vi "Process.vi"(8 "error in (no error)":errorcluster, 10 "Event Registration Refnum":refnum<event-registration>, 11 "Test Manager":refnum<class "Basic Test Manager.lvclass">) -> (0 "error out":errorcluster, 3 "Test Manager out":refnum<class "Basic Test Manager.lvclass">)   [LabVIEW 2020, in "Caraya.lvlib" / "Basic Test Manager.lvclass"]
uses:
  Basic Test Manager.lvclass
  Basic Test Manager.lvclass/Basic Test Manager.ctl
  Test Event Storage/Test Event Storage.lvclass
  Test State.ctl
  <vilib>/picture/picture.llb/imagedata.ctl
  Test Result/Test Registration Data.ctl
  Test Result/Test Result.lvclass
  Caraya.lvlib
  Tree Symbol.ctl
  <vilib>/Platform/browser.llb/Open URL in Default Browser (string).vi
  Test Report/Test Report.lvclass
  Test Report.JUnit/Test Report.JUnit.lvclass
  Test Report.Default/Test Report.Default.lvclass
  <userlib>/_OpenG.lib/file/file.llb/openg_file.lvlib
  <userlib>/_OpenG.lib/file/file.llb/Strip Path Extension - String__ogtk.vi
  Test Manager Message/TestManagerMsg.lvclass
  Test Manager Message Assertion/TestManagerMsg.Assertion.lvclass
  Test Manager Message Verbose/TestManagerMsg.Verbose.lvclass
  Test Manager Message KVP/TestManagerMsg.KVP.lvclass
  Test Manager Message Measurement/TestManagerMsg.Measurement.lvclass
  Test Manager Message Test/TestManagerMsg.Test.lvclass
  Test Manager Message Complete Suite/TestManagerMsg.CompleteSuite.lvclass
  Test Report.Event/Test Report.Event.lvclass
  Test Result/Test Node (Extended).ctl
  C:/projects/caraya/src/classes/Test Manager Message/TestManagerMsg.lvclass
  C:/projects/caraya/src/classes/Test Report/Test Report.lvclass
  UI Tab -- enum.ctl
panel:
  out "Processing Time (s)":dbl
  in  "Unknow":bool caption="Unknown"
  out "Pass":bool caption="Passed"
  in  "Fail":bool caption="Failed"
  in  "Hide Passed Tests Checkbox":bool
  out "Error String":string="0 Errors"
  out "Fail String":string="0 Failed"
  out "Pass String":string="0 Passed"
  out "Skip String":string="0 Skipped"
  out "Unknown String":string="0 Unknowns"
  in  "Tab":T1
  out "Report":string
  in  "Tests Tree":string(tree)
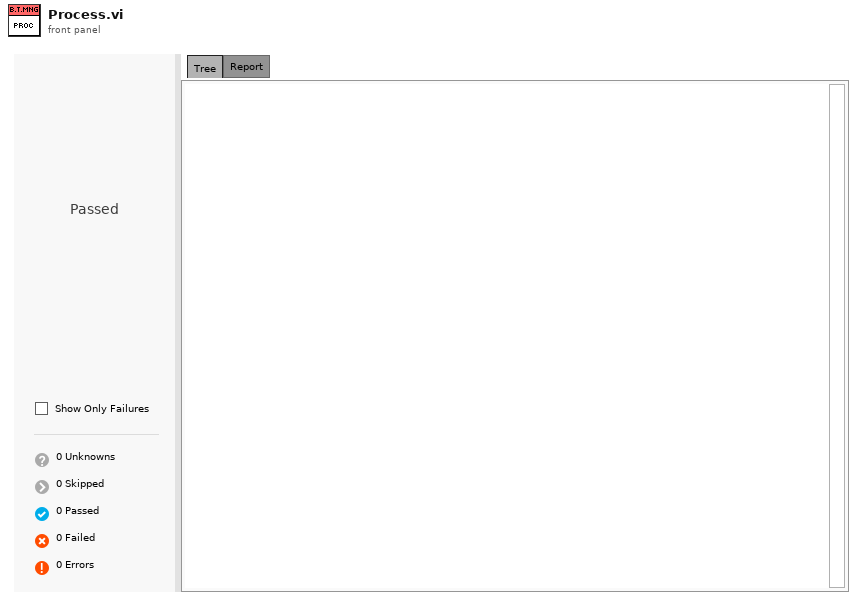
[diagram p1: front panel]
types:
  T1 = typedef "Caraya.lvlib/Basic Test Manager.lvclass/UI Tab -- enum.ctl" = enum32{"Tree", "Report"}
  T2 = enum32{"invalid app kind", "Development System", "Run Time System", "Student Edition", "Embedded LabVIEW", "Evaluation", "Custom"}
  T3 = typedef "Caraya.lvlib/Test Result.lvclass/Test Node (Extended).ctl" = cluster{"Test Registration":T4, "Defined":bool, "Passed":bool, "properties":variant}
  T4 = typedef "Caraya.lvlib/Test Result.lvclass/Test Registration Data.ctl" = cluster{"Name":string, "Call Chain":string[], "Time Stamp":timestamp, "Test ID":string, "Caller ID":string}
  T5 = enum32{"Page Enabled", "Page Disabled", "Page Disabled & Grayed"}
  T6 = enum32{"Invalid", "Standard", "Closed", "Hidden", "Minimized", "Maximized"}
  T7 = typedef "Caraya.lvlib/Basic Test Manager.lvclass/Test State.ctl" = enum16{"Empty", "Unknown", "Fail", "Pass", "Skip", "Error"}
  T8 = cluster{"Core":cluster{"Current VI Reference":refnum<vi>, "Close Panel on Exit?":bool}, "State":T7, "Storage":refnum<class "Test Event Storage.lvclass">, "Argument":variant, "Final State":T7, "Complete":bool, "Last Update":u32, "Running":bool, "Hide Passed Tests":bool, "final error":errorcluster, "Update Delay":u32, "Message":refnum<class "TestManagerMsg.lvclass">, "Tab":T1, "Report Event":refnum<user-event>, "Start Time":timestamp}
  T9 = typedef "LVPoint32TypeDef.ctl" = cluster{"Horizontal":i32, "Vertical":i32}
  T10 = cluster{"Current VI Reference":refnum<vi>, "Close Panel on Exit?":bool}
  T11 = cluster{"Event Registration Refnum":refnum<event-registration>, "local":refnum<event-registration>}
  T12 = typedef "imagedata.ctl" = cluster{"image type":i32, "image depth":i32, "image":u8[], "mask":u8[], "colors":u32[], "Rectangle":cluster{"left":i16, "top":i16, "right":i16, "bottom":i16}}
  T13 = typedef "Caraya.lvlib/Basic Test Manager.lvclass/Tree Symbol.ctl" = enum16{"Empty", "Unknown", "Fail", "Pass", "Skip", "Error", "Fail Node", "Pass Node"}
  T14 = typedef "Caraya.lvlib/Test Result.lvclass/Assert Event Data (Extended).ctl" = cluster{"name":string, "passed":bool, "call-chain":string[], "test-error":errorcluster, "timestamp":timestamp, "assert-id":string, "test-id":string, "time":dbl, "message":string, "properties":variant, "measurements":variant, "user-defined":variant}
  T15 = typedef "Caraya.lvlib/Test Result.lvclass/Test Node.ctl" = cluster{"Test Registration":T4, "Defined":bool, "Passed":bool}
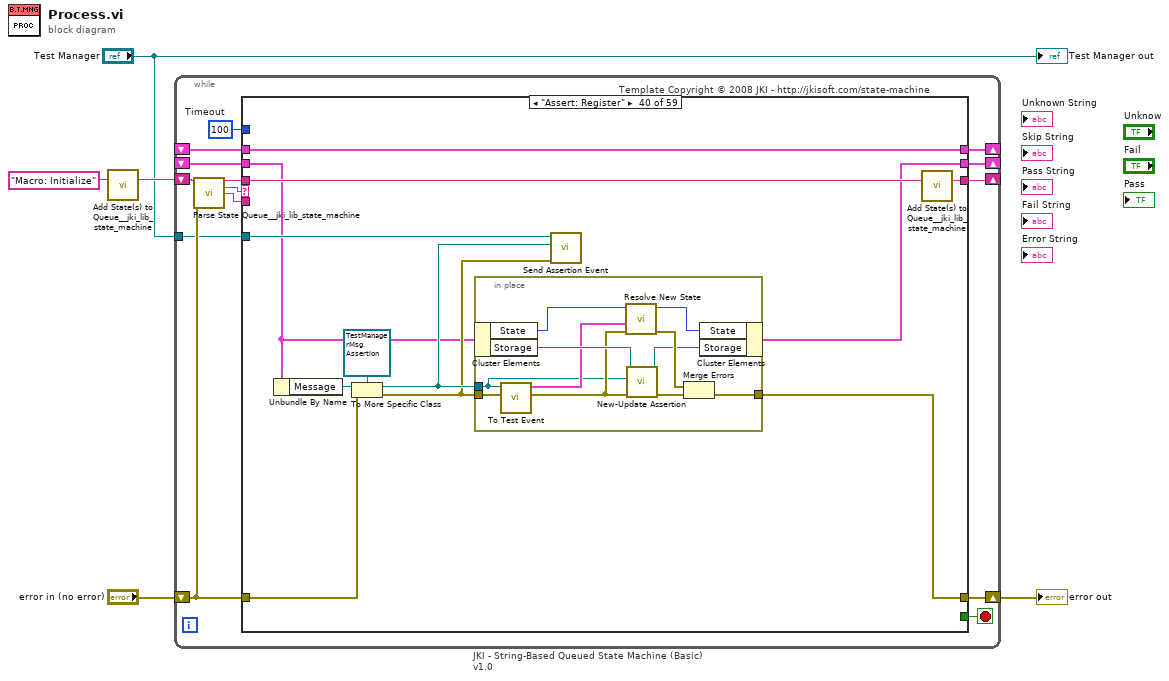
[diagram p0: block diagram]
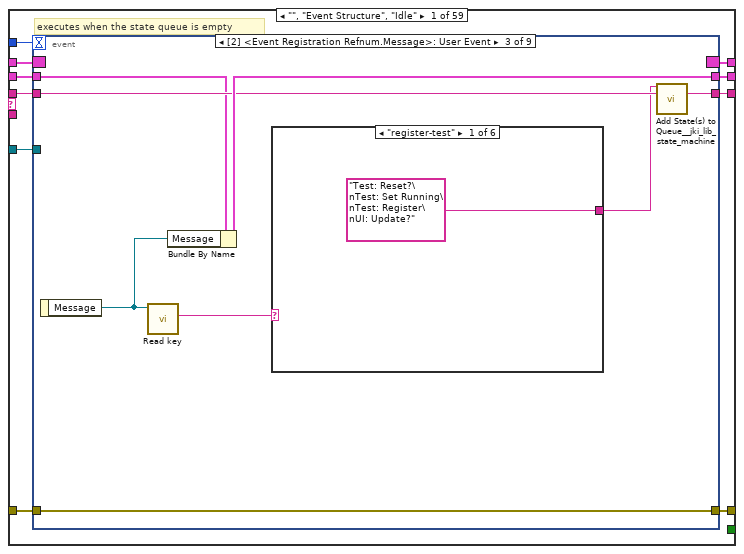
[diagram p2: hidden frame]
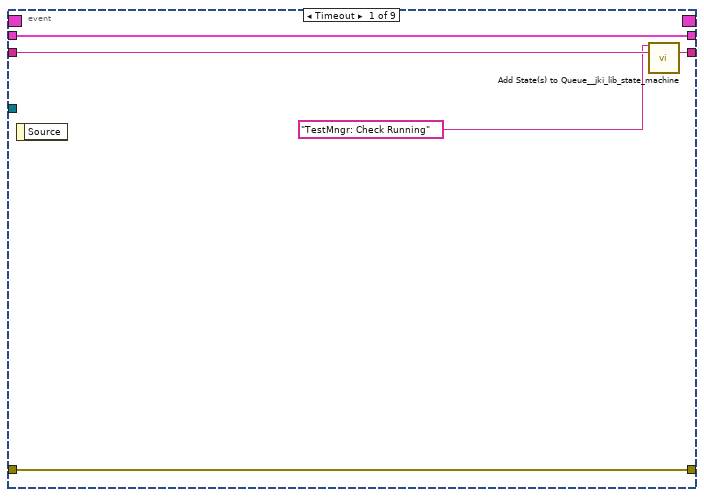
[diagram p3: hidden frame]
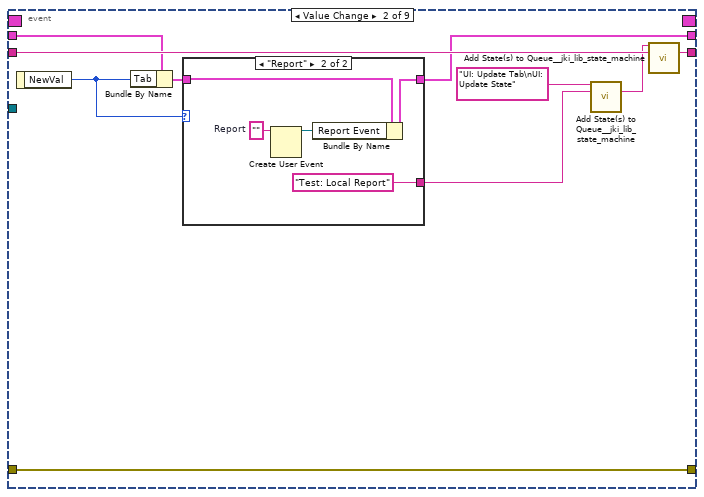
[diagram p4: hidden frame]
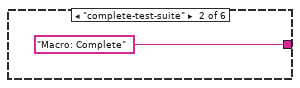
[diagram p6: hidden frame]
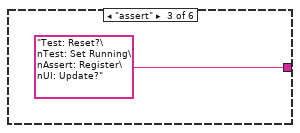
[diagram p7: hidden frame]
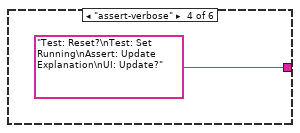
[diagram p8: hidden frame]
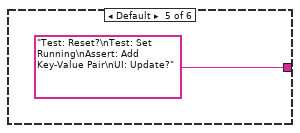
[diagram p9: hidden frame]
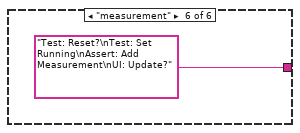
[diagram p10: hidden frame]
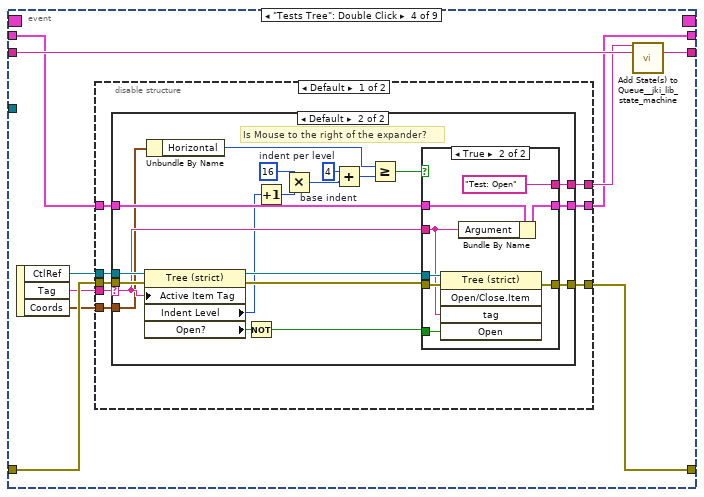
[diagram p11: hidden frame]
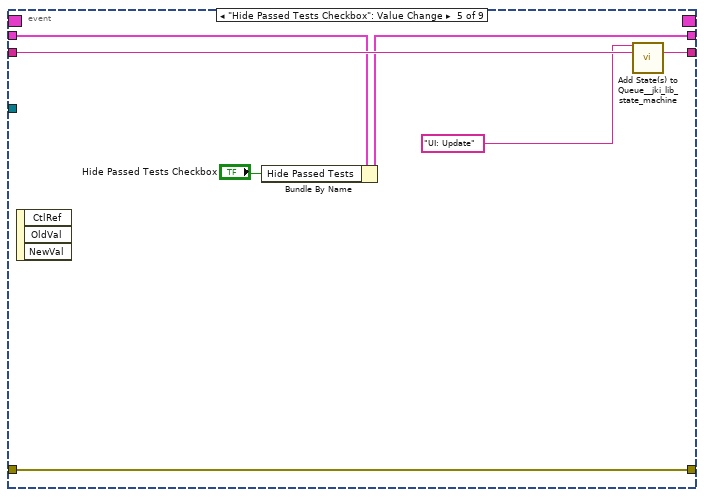
[diagram p15: hidden frame]
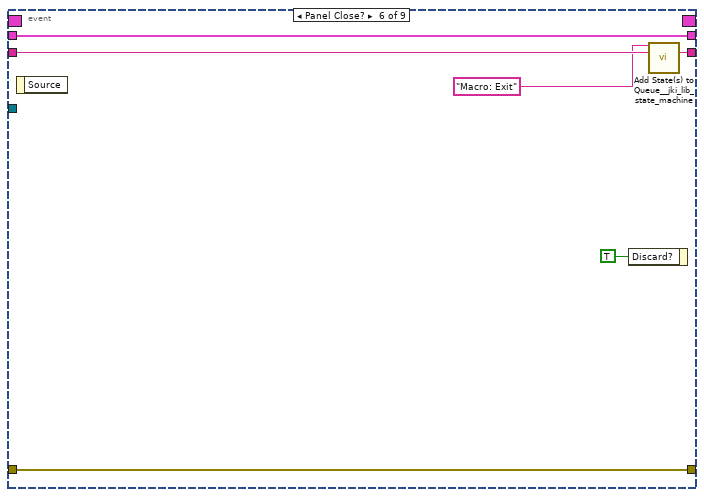
[diagram p16: hidden frame]
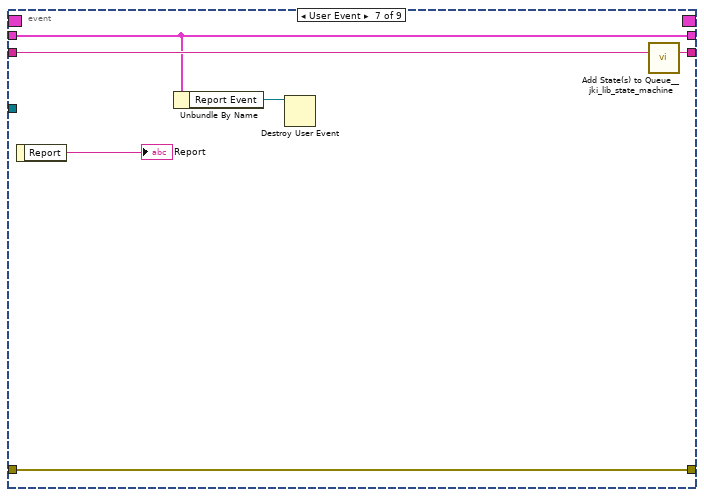
[diagram p17: hidden frame]
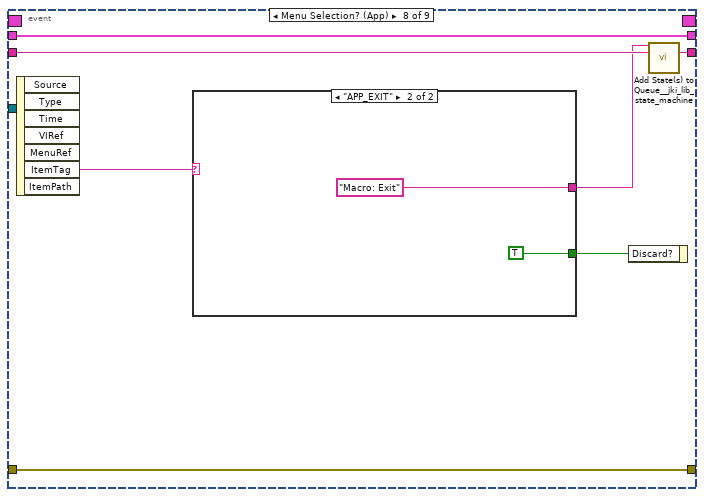
[diagram p18: hidden frame]
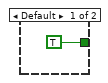
[diagram p19: hidden frame]
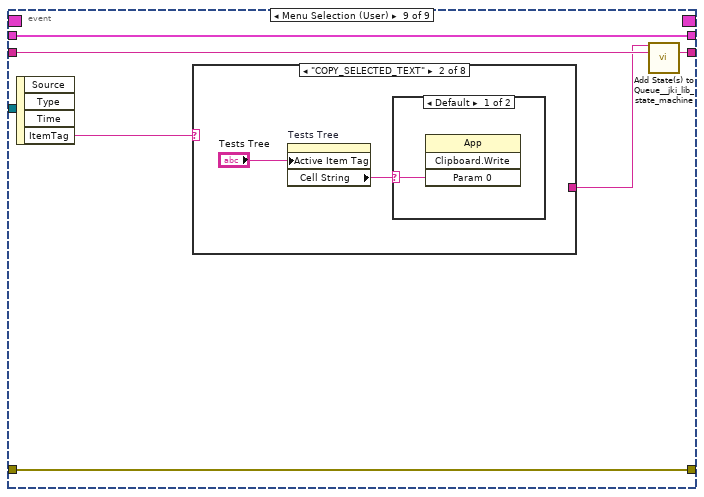
[diagram p20: hidden frame]
diagram:
  n1 = call <vilib>:"Add State(s) to Queue__jki_lib_state_machine.vi"("State(s) in (\"\")"="Macro: Initialize") -> ("States Out"=w5:string)  [unwired: 14 in]
  n2 = while "JKI - String-Based Queued State Machine (Basic) v1.0" {
    shift-right: [w12] -> _
    shift-left: _ -> [w11]
    shift-right: [w15] -> w1
    shift-left: "error in (no error)" -> [w9]
    shift-right: [w14] -> _
    shift-left: w5 -> [w16]
    tunnel: "Test Manager" -> [w7]
    shift-right: [w6] -> _
    shift-left: _ -> [w8]
    stop <- w13 stop-if-true
    w10 = 100  # Timeout
    # "Template Copyright © 2008 JKI - http://jkisoft.com/state-machine"
    n3 = call <vilib>:"Parse State Queue__jki_lib_state_machine.vi"("State Queue"=w16, "Error In (no error)"=w9) -> ("Remaining States"=w18:string, "Current State"=w19:string, "Arguments"=w17:string)  [unwired: 11 in]
    n4 = case shown="\"Assert: Register\"" w19 {
      selector: w19 -> [_ _ w168 _ _ _ _ _ _ _ _ _ _ _ _ _ _ _ _ _ _ _ _ _ _ _ _ _ _ _ _ _ _ _ _ _ _ _ _ _ _ _ _ _ _ _ _ _ _ _ _ _ _ _ _ _ _ _ _]
      tunnel: w18 -> [w29 w165 w172 w190 w202 w213 w219 w224 w240 w251 w256 w265 w270 w277 w283 w296 w304 w316 w329 w339 w345 w357 w367 w385 w391 w411 w463 w505 w539 w556 w574 w607 w613 w619 w625 w631 w637 w649 w654 w666 w687 w712 w734 w755 w771 w776 w796 w807 w809 w856 w883 w892 w899 w909 w921 w943 w957 w987 w1035]
      tunnel: w17 -> [_ _ _ _ _ _ _ _ _ _ _ _ _ _ _ _ _ _ _ _ _ _ _ _ _ _ _ _ w534 w553 w569 _ _ _ _ _ _ _ _ _ _ _ _ _ _ _ _ _ _ _ _ _ _ _ _ _ _ w962 _]
      tunnel: w11 -> [w27 w162 w170 w181 w195 w211 w216 w221 _ w246 w253 w258 w267 w273 w281 w293 w302 w313 w318 w332 w343 w355 w365 w377 w389 w409 w458 w502 w537 w551 w570 w604 w610 w616 w622 w628 w634 w646 w651 w655 w683 w709 w731 w752 w763 w773 w790 w805 w810 w849 w878 w888 w896 w903 w917 w933 w955 w984 w1031]
      tunnel: [w26 w163 w174 w187 errorcluster {"status"=FALSE, "code"=0, "source"=""} ("error out") w208 w215 w222 w242 w247 w254 w263 w268 w275 w279 w294 w300 w314 w327 w337 w341 w354 w363 w383 w388 w408 w459 w503 w535 w552 w571 w605 w611 w617 w623 w629 w635 w647 w652 w663 w678 w702 w735 w753 w767 w774 w794 w802 w811 w845 w881 w890 w897 w907 w918 w931 w948 w985 w1033] -> w15
      tunnel: w9 -> [w25 w163 w173 w187 w198 w208 w215 w222 w242 w248 w254 w263 w268 w275 w280 w294 w301 w314 w327 w337 w342 w353 w364 w383 w387 w407 w461 w503 w536 w549 w572 w605 w611 w617 w623 w629 w635 w647 w652 w660 w684 w704 w728 w753 w768 w774 w793 w803 w813 w846 w881 w890 w897 w907 w919 w928 w952 w977 w1033]
      tunnel: [w28 w164 w171 w189 w201 w212 w218 w223 w244 w250 w255 w264 w269 w276 w282 w295 w303 w315 w328 w338 w344 w356 w366 w384 w390 w410 w462 w504 w538 w555 w573 w606 w612 w618 w624 w630 w636 w648 w653 w665 w688 w714 w737 w754 w770 w775 w795 w806 w814 w855 w882 w891 w898 w908 w920 w942 w956 w986 w1034] -> w14
      tunnel: [_ _ _ _ _ _ TRUE _ _ _ _ _ _ _ _ _ _ _ _ _ _ _ _ _ _ _ _ _ _ _ _ _ _ _ _ _ _ _ _ _ _ _ _ _ _ _ _ _ _ _ _ _ _ _ _ _ _ _ _] -> w13
      tunnel: [w24 w162 w170 w188 w196 w210 w216 w221 w243 w246 w253 w258 w267 w273 w281 w293 w302 w313 w318 w332 w343 w355 w365 w382 w389 w409 w458 w502 w537 w551 w570 w604 w610 w616 w622 w628 w634 w646 w651 w664 w677 w713 w736 w752 w763 w773 w791 w805 w810 w849 w880 w888 w895 w903 w917 w933 w955 w984 w1032] -> w12
      tunnel: w10 -> [w23 _ _ _ _ _ _ _ _ _ _ _ _ _ _ _ _ _ _ _ _ _ _ _ _ _ _ _ _ _ _ _ _ _ _ _ _ _ _ _ _ _ _ _ _ _ _ _ _ _ _ _ _ _ _ _ _ _ _]
      tunnel: w8 -> [w21 w161 w166 w178 w191 w207 w214 w220 w227 w245 w252 _ w266 w271 w278 w289 w298 w311 w317 w330 w340 w352 w362 w373 w386 w406 w457 w501 w533 w548 w568 w603 w608 w614 w620 w626 w632 w638 w650 w659 w682 w705 w726 w751 w756 w772 w785 w797 w808 w844 w873 w884 w893 w900 w911 w939 w944 w959 w1020]
      tunnel: w7 -> [w22 _ _ _ _ _ _ _ _ _ _ _ _ _ _ _ _ _ _ w333 _ _ _ _ _ _ _ _ _ _ _ _ _ _ _ _ _ _ _ w658 w681 w711 w733 _ _ _ w784 _ w812 _ _ _ _ w904 w915 w927 w953 w970 _]
      tunnel: [w20 w161 w166 w178 w191 w207 w214 w220 w227 w245 w252 w261 w266 w271 w278 w289 w298 w311 w317 w330 w340 w352 w362 w373 w386 w406 w457 w501 w533 w548 w568 w603 w608 w614 w620 w626 w632 w638 w650 w659 w682 w705 w726 w751 w756 w772 w785 w797 w808 w844 w873 w884 w893 w900 w911 w939 w944 w959 w1020] -> w6
      frame "", "Event Structure", "Idle" {
        # "executes when the state queue is empty"
        n5 = event shown="[2] <Event Registration Refnum.Message>: User Event" {
          selector: w21 -> [_ _ _ _ _ _ _ _ _]
          dyn-events: [_ _ _ _ _ _ _ _ _] -> w20
          timeout: w23 -> [_ _ _ _ _ _ _ _ _]
          tunnel: w29 -> [w34 w44 w54 w73 w122 w129 w135 w142 w151]
          tunnel: [w33 w43 w55 w74 w123 w128 w134 w141 w150] -> w28
          tunnel: w27 -> [w31 w41 w52 w68 w119 w126 w131 w139 w148]
          tunnel: [w32 w42 w58 w71 w120 w127 w133 w140 w149] -> w26
          tunnel: w25 -> [w32 w42 w58 w70 w120 w127 w133 w140 w149]
          tunnel: [w31 w35 w56 w69 w118 w126 w131 w139 w148] -> w24
          tunnel: w22 -> [_ _ _ _ _ _ _ _ _]
          event Timeout {
            n6 = event-data() -> ()  [unwired: 1 in, 1 out]
            n7 = call <vilib>:"Add State(s) to Queue__jki_lib_state_machine.vi"("State(s) in Front (\"\")"="TestMngr: Check Running", "State(s) in (\"\")"=w34) -> ("States Out"=w33:string)  [unwired: 13 in]
          }
          event Value Change {
            n8 = event-data() -> ("NewVal"=w38:T1)  [unwired: 1 in]
            n9 = Bundle By Name(cluster=w41, "Tab"=w38) -> (w36:T8)
            n10 = case shown="\"Report\"" w38 {
              tunnel: [_ "Test: Local Report"] -> w37
              tunnel: w36 -> [w45 w49]
              tunnel: [w45 w48] -> w35
              frame Default {
              }
              frame "Report" {
                w47 = ""  # Report
                n11 = Create User Event(user event datatype=w47) -> (user event=w46:refnum<user-event>)  [unwired: 1 in, 1 out]
                n12 = Bundle By Name(cluster=w49, "Report Event"=w46) -> (w48:T8)
              }
            }
            n13 = call <vilib>:"Add State(s) to Queue__jki_lib_state_machine.vi"("State(s) in Front (\"\")"="UI: Update Tab\nUI: Update State", "State(s) in (\"\")"=w37) -> ("States Out"=w39:string)  [unwired: 13 in]
            n14 = call <vilib>:"Add State(s) to Queue__jki_lib_state_machine.vi"("State(s) in Front (\"\")"=w39, "State(s) in (\"\")"=w44) -> ("States Out"=w43:string)  [unwired: 13 in]
          }
          event User Event {
            n15 = event-data() -> ("Message"=w57:refnum<class "TestManagerMsg.lvclass">)  [unwired: 1 in]
            n16 = call "Read key.vi"("TestManagerMsg in"=w57) -> ("key"=w51:string)  [unwired: 9 in, 1 out]
            n17 = Bundle By Name(cluster=w52, "Message"=w57) -> (w56:T8)
            n18 = case shown="\"register-test\"" w51 {
              tunnel: ["Test: Reset?\nTest: Set Running\nTest: Register\nUI: Update?" "Macro: Complete" "Test: Reset?\nTest: Set Running\nAssert: Register\nUI: Update?" "Test: Reset?\nTest: Set Running\nAssert: Update Explanation\nUI: Update?" "Test: Reset?\nTest: Set Running\nAssert: Add Key-Value Pair\nUI: Update?" "Test: Reset?\nTest: Set Running\nAssert: Add Measurement\nUI: Update?"] -> w53
              frame "register-test" {
              }
              frame "complete-test-suite" {
              }
              frame "assert" {
              }
              frame "assert-verbose" {
              }
              frame Default {
              }
              frame "measurement" {
              }
            }
            n19 = call <vilib>:"Add State(s) to Queue__jki_lib_state_machine.vi"("State(s) in Front (\"\")"=w53, "State(s) in (\"\")"=w54) -> ("States Out"=w55:string)  [unwired: 13 in]
          }
          event "Tests Tree": Double Click {
            n20 = event-data() -> ("CtlRef"=w66:refnum<vi>, "Tag"=w67:string, "Coords"=w65:T9)  [unwired: 1 in]
            n21 = disable-structure shown="Default" {
              disable-tunnel: [w82 _] -> w72
              disable-tunnel: [w81 w115] -> w71
              disable-tunnel: w70 -> [w80 w115]
              disable-tunnel: [w79 w116] -> w69
              disable-tunnel: w68 -> [w78 w116]
              disable-tunnel: w67 -> [w77 _]
              disable-tunnel: w66 -> [w76 _]
              disable-tunnel: w65 -> [w75 _]
              frame condition #0 (active) {
                n22 = case shown="Default" w77 {
                  selector: w77 -> [_ w99]
                  tunnel: [_ w104] -> w82
                  tunnel: [w83 w86] -> w81
                  tunnel: w76 -> [_ w103]
                  tunnel: w80 -> [w83 w102]
                  tunnel: w78 -> [w84 w101]
                  tunnel: [w84 w100] -> w79
                  tunnel: w75 -> [_ w90]
                  frame "" {
                  }
                  frame Default {
                    w93 = 16  # indent per level
                    w92 = 4  # base indent
                    # "Is Mouse to the right of the expander?"
                    n23 = property class="Tree (strict)"(reference=w103, error in=w102, "Active Item Tag"=w99) -> (reference out=w98:refnum<vi>, error out=w97:errorcluster, "Indent Level"=w95:i32, "Open?"=w96:bool)
                    n24 = Unbundle By Name(w90) -> ("Horizontal"=w88:i32)
                    n25 = Not(x=w96) -> (.not. x?=w85:bool)
                    n26 = Increment(x=w95) -> (x+1=w94:i32)
                    n27 = Multiply(x=w93, y=w94) -> (x*y=w91:i32)
                    n28 = Add(x=w92, y=w91) -> (x+y=w87:i32)
                    n29 = Greater Or Equal?(x=w88, y=w87) -> (x >= y?=w89:bool)
                    n30 = case shown="True" w89 {
                      tunnel: [_ "Test: Open" ("State(s) in Front (\"\")")] -> w104
                      tunnel: w101 -> [w106 w113]
                      tunnel: [w106 w112] -> w100
                      tunnel: w99 -> [_ w108]
                      tunnel: [w105 w110] -> w86
                      tunnel: w98 -> [_ w109]
                      tunnel: w97 -> [w105 w111]
                      tunnel: w85 -> [_ w107]
                      frame False {
                      }
                      frame True {
                        n31 = invoke class="Tree (strict)" method="Open/Close.Item"(reference=w109, error in=w111, "tag"=w108, "Open"=w107) -> (error out=w110:errorcluster)  [unwired: 1 in, 4 out]
                        n32 = Bundle By Name(cluster=w113, "Argument"=w108) -> (w112:T8)
                      }
                    }
                  }
                }
              }
              frame condition #1 {
              }
            }
            n33 = call <vilib>:"Add State(s) to Queue__jki_lib_state_machine.vi"("State(s) in Front (\"\")"=w72, "State(s) in (\"\")"=w73) -> ("States Out"=w74:string)  [unwired: 13 in]
          }
          event "Hide Passed Tests Checkbox": Value Change {
            n34 = event-data() -> ()  [unwired: 1 in, 3 out]
            n35 = Bundle By Name(cluster=w119, "Hide Passed Tests"="Hide Passed Tests Checkbox") -> (w118:T8)
            n36 = call <vilib>:"Add State(s) to Queue__jki_lib_state_machine.vi"("State(s) in Front (\"\")"="UI: Update" ("State(s) in Front (\"\")"), "State(s) in (\"\")"=w122) -> ("States Out"=w123:string)  [unwired: 13 in]
          }
          event Panel Close? {
            n37 = event-data() -> ()  [unwired: 1 in, 1 out]
            n38 = event-data("Discard?"=TRUE) -> ()  [unwired: 1 in, 1 out]
            n39 = call <vilib>:"Add State(s) to Queue__jki_lib_state_machine.vi"("State(s) in Front (\"\")"="Macro: Exit", "State(s) in (\"\")"=w129) -> ("States Out"=w128:string)  [unwired: 13 in]
          }
          event User Event {
            n40 = event-data() -> ("Report"=→"Report":string)  [unwired: 1 in]
            n41 = Unbundle By Name(w131) -> ("Report Event"=w130:refnum<user-event>)
            n42 = Destroy User Event(user event=w130) -> ()  [unwired: 1 in, 1 out]
            n43 = call <vilib>:"Add State(s) to Queue__jki_lib_state_machine.vi"("State(s) in (\"\")"=w135) -> ("States Out"=w134:string)  [unwired: 14 in]
          }
          event Menu Selection? (App) {
            n44 = event-data() -> ("ItemTag"=w137:string)  [unwired: 1 in, 6 out]
            n45 = case shown="\"APP_EXIT\"" w137 {
              tunnel: [_ "Macro: Exit"] -> w138
              tunnel: [TRUE TRUE] -> w136
              frame Default {
              }
              frame "APP_EXIT" {
              }
            }
            n46 = event-data("Discard?"=w136) -> ()  [unwired: 1 in, 1 out]
            n47 = call <vilib>:"Add State(s) to Queue__jki_lib_state_machine.vi"("State(s) in Front (\"\")"=w138, "State(s) in (\"\")"=w142) -> ("States Out"=w141:string)  [unwired: 13 in]
          }
          event Menu Selection (User) {
            n48 = event-data() -> ("ItemTag"=w146:string)  [unwired: 1 in, 3 out]
            n49 = case shown="\"COPY_SELECTED_TEXT\"" w146 {
              tunnel: [_ _ "Macro: Export" "Macro: Export JUnit" "Macro: Rerun" "UI: About" "UI: Homepage" "Macro: Exit"] -> w147
              frame Default {
              }
              frame "COPY_SELECTED_TEXT" {
                n50 = property on="Tests Tree" class="Tree (strict)"("Active Item Tag"="Tests Tree") -> ("Cell String"=w152:string)  [unwired: 2 in, 2 out]
                n51 = case shown="Default" w152 {
                  selector: w152 -> [w154 _]
                  frame Default {
                    n52 = invoke class="App" method="Clipboard.Write"("Param 0"=w154) -> ()  [unwired: 3 in, 4 out]
                  }
                  frame "" {
                  }
                }
              }
              frame "FILE_EXPORT" {
              }
              frame "FILE_EXPORT_JUNIT" {
              }
              frame "TEST_RERUN" {
              }
              frame "HELP_ABOUT" {
              }
              frame "HOME_PAGE" {
              }
              frame "FILE_CLOSE" {
              }
            }
            n53 = call <vilib>:"Add State(s) to Queue__jki_lib_state_machine.vi"("State(s) in Front (\"\")"=w147, "State(s) in (\"\")"=w151) -> ("States Out"=w150:string)  [unwired: 13 in]
          }
        }
      }
      frame "---------- Core ----------" {
        # "Do not put any code in this frame.\n(it is a separator no-op)"
        n54 = call <vilib>:"Add State(s) to Queue__jki_lib_state_machine.vi"("State(s) in (\"\")"=w165) -> ("States Out"=w164:string)  [unwired: 14 in]
      }
      frame Default {
        # "Current State"
        # "Do not delete, rename, or modify this frame.\n(this is used to capture unhandled states and typos)"
        # "Handle mistyped state name (developer tool)"
        n55 = Format Into String(format string="Software Exception: Unhandled State \"%s\"." ("message"), error in=w173, w168) -> (resulting string=w176:string, error out=w175:errorcluster)  [unwired: 1 in]
        n56 = call <vilib>:"Error Cluster From Error Code.vi"("show call chain? (False)"=TRUE, "error in (no error)"=w175, "error message (\"\")"=w176, "error code (0)"=7000) -> ("error out"=w174:errorcluster)  [unwired: 5 in]
        n57 = call <vilib>:"Add State(s) to Queue__jki_lib_state_machine.vi"("State(s) in (\"\")"=w172) -> ("States Out"=w171:string)  [unwired: 14 in]
      }
      frame "Initialize Core Data" {
        # "Do not delete, rename, or modify this frame.\n(this is used to determine panel behavior on exit)"
        # "originally closed?"
        # "exe?"
        # "If panel starts closed or is an EXE, then close it when we exit"
        n58 = stacked-sequence {
          frame #0 {
            # "Do not delete. This reference forces\nFront Panel in memory in EXE."
            n59 = control-ref of="Test Manager"() -> ()  [unwired: 1 out]
          }
        }
        n60 = property class="VI"() -> ("Front Panel.Open"=w186:bool)  [unwired: 2 in, 2 out]
        n61 = property class="App"() -> ("App.Kind"=w185:T2)  [unwired: 2 in, 2 out]
        n62 = control-ref of="Current VI Reference"() -> (w179:refnum<vi>)
        n63 = Not(x=w186) -> (.not. x?=w183:bool)
        n64 = Equal?(x=w185, y=T2."Run Time System" ("Application:Kind")) -> (x = y?=w182:bool)
        n65 = Or(x=w183, y=w182) -> (x .or. y?=w180:bool)
        n66 = Bundle By Name(cluster=w181, "Core.Current VI Reference"=w179, "Core.Close Panel on Exit?"=w180) -> (w188:T8)
        n67 = call <vilib>:"Add State(s) to Queue__jki_lib_state_machine.vi"("State(s) in (\"\")"=w190) -> ("States Out"=w189:string)  [unwired: 14 in]
      }
      frame "Error Handler" {
        # "Clear error"
        # "Handle any errors here.\nYou can also output any states to clean-up after errors occur"
        n68 = Unbundle By Name(w198) -> ("code"=w199:i32)
        n69 = case shown="Default" w199 {
          tunnel: w198 -> [w203 w204 w206]
          tunnel: [w203 w204 w205] -> w193
          frame 7000..7999 {
            # "All Caraya Error range"
          }
          frame 1 {
          }
          frame Default {
            # "Unhandled Error -- Display it"
            n70 = call <vilib>:"General Error Handler.vi"("error in (no error)"=w206) -> ("error out"=w205:errorcluster)  [unwired: 10 in, 4 out]
          }
        }
        n71 = Unbundle By Name(w195) -> ("final error"=w194:errorcluster)
        n72 = Merge Errors(w194, w193) -> (w192:errorcluster)
        n73 = Bundle By Name(cluster=w195, "final error"=w192) -> (w196:T8)
        n74 = call <vilib>:"Add State(s) to Queue__jki_lib_state_machine.vi"("State(s) in Front (\"\")"="/* Post Error States", "State(s) in (\"\")"=w202) -> ("States Out"=w201:string)  [unwired: 13 in]
      }
      frame "Reset Final Error" {
        # "Clear error"
        n75 = Bundle By Name(cluster=w211, "final error"=errorcluster {"status"=FALSE, "code"=0, "source"=""} ("error out")) -> (w210:T8)
        n76 = call <vilib>:"Add State(s) to Queue__jki_lib_state_machine.vi"("State(s) in (\"\")"=w213) -> ("States Out"=w212:string)  [unwired: 14 in]
      }
      frame "Exit" {
        # "Do not put any code in this frame.\n(No errors that occur here will be handled.)"
        n77 = call <vilib>:"Add State(s) to Queue__jki_lib_state_machine.vi"("State(s) in (\"\")"=w219) -> ("States Out"=w218:string)  [unwired: 14 in]
      }
      frame "---------- Data ----------" {
        # "Do not put any code in this frame.\n(It is a separator no-op. You can make a copy of this frame to create a new Data frame)"
        n78 = call <vilib>:"Add State(s) to Queue__jki_lib_state_machine.vi"("State(s) in (\"\")"=w224) -> ("States Out"=w223:string)  [unwired: 14 in]
      }
      frame "Data: Initialize" {
        w225 = timestamp(0 s since 1904-01-01)  # Start Time
        w226 = refnum<user-event> refnum  # Report Event
        w229 = refnum<class "TestManagerMsg.lvclass"> refnum  # Message
        w230 = u32 100  # Update Delay
        w231 = errorcluster {"status"=FALSE, "code"=0, "source"=""}  # final error
        w232 = FALSE  # Hide Passed Tests
        w233 = FALSE  # Running
        w234 = u32 0  # Last Update
        w235 = FALSE  # Complete
        w236 = Test_State."Unknown"  # Final State
        w237 = variant  # Argument
        w239 = Test_State."Unknown"  # State
        w238 = refnum<class "Test Event Storage.lvclass"> refnum  # Storage
        w241 = T10 {"Current VI Reference"=refnum, "Close Panel on Exit?"=FALSE}  # Core
        # "Initialize the shift-register data, here.\n(data names are defined by what you wire into the bundle function)"
        n79 = Bundle("Core"=w241, "State"=w239, "Storage"=w238, "Argument"=w237, "Final State"=w236, "Complete"=w235, "Last Update"=w234, "Running"=w233, "Hide Passed Tests"=w232, "final error"=w231, "Update Delay"=w230, "Message"=w229, "Tab"="Tab", "Report Event"=w226, "Start Time"=w225) -> (w243:T8)  [unwired: 1 in]
        n80 = call <vilib>:"Add State(s) to Queue__jki_lib_state_machine.vi"("State(s) in (\"\")"=w240) -> ("States Out"=w244:string)  [unwired: 14 in]
      }
      frame "Data: Cleanup" {
        # "Cleanup any data and references, here.\n(this is called automatically, by the Macro: Exit)"
        n81 = Unbundle By Name(w246) -> ("Core.Current VI Reference"=w249:refnum<vi>)
        n82 = Close Reference(reference=w249, error in (no error)=w248) -> (error out=w247:errorcluster)
        n83 = call <vilib>:"Add State(s) to Queue__jki_lib_state_machine.vi"("State(s) in (\"\")"=w251) -> ("States Out"=w250:string)  [unwired: 14 in]
      }
      frame "---------- Event ----------" {
        # "Do not put any code in this frame.\n(It is a separator no-op. You can make a copy of this frame to create a new UI frame)"
        n84 = call <vilib>:"Add State(s) to Queue__jki_lib_state_machine.vi"("State(s) in (\"\")"=w256) -> ("States Out"=w255:string)  [unwired: 14 in]
      }
      frame "Event: Register" {
        w260 = refnum<event-registration> refnum  # local
        n85 = Unbundle By Name(w258) -> ("Report Event"=w257:refnum<user-event>)
        n86 = register-events(reference=w260, w257) -> (reference out=w262:refnum<event-registration>)  [unwired: 1 in, 1 out]
        n87 = Bundle("Event Registration Refnum"="Event Registration Refnum", "local"=w262) -> (w261:T11)  [unwired: 1 in]
        n88 = call <vilib>:"Add State(s) to Queue__jki_lib_state_machine.vi"("State(s) in (\"\")"=w265) -> ("States Out"=w264:string)  [unwired: 14 in]
      }
      frame "---------- UI ----------" {
        # "Do not put any code in this frame.\n(It is a separator no-op. You can make a copy of this frame to create a new UI frame)"
        n89 = call <vilib>:"Add State(s) to Queue__jki_lib_state_machine.vi"("State(s) in (\"\")"=w270) -> ("States Out"=w269:string)  [unwired: 14 in]
      }
      frame "UI: Initialize" {
        # "Initialize the User Interface, here.\n(this is called automatically, by the Macro: Init)"
        n90 = Unbundle By Name(w273) -> ("Hide Passed Tests"=w272:bool)
        n91 = local write "Hide Passed Tests Checkbox"(w272) -> ()
        n92 = call <vilib>:"Add State(s) to Queue__jki_lib_state_machine.vi"("State(s) in Front (\"\")"="//UI: Defer Updates >> True\nUI: Initialize Icons\nUI: Clear\nUI: Update Title\nUI: Update State\nUI: Set Last Update\n//UI: Defer Updates >> False", "State(s) in (\"\")"=w277) -> ("States Out"=w276:string)  [unwired: 13 in]
      }
      frame "UI: Update Title" {
        n93 = disable-structure shown="Default" {
          disable-tunnel: w280 -> [w285 w288]
          disable-tunnel: [w284 w288] -> w279
          frame condition #0 (active) {
            n94 = control-ref of="This VI"() -> (w287:refnum<vi>)
            n95 = call "Get Library Info.vi"("error in (no error)"=w285) -> ("error out"=w284:errorcluster, "Name"=w286:string)  [unwired: 6 in, 3 out]
            n96 = property class="VI"(reference=w287, "Front Panel.Title"=w286) -> ()  [unwired: 1 in, 2 out]
          }
          frame condition #1 {
          }
        }
        n97 = call <vilib>:"Add State(s) to Queue__jki_lib_state_machine.vi"("State(s) in (\"\")"=w283) -> ("States Out"=w282:string)  [unwired: 14 in]
      }
      frame "UI: Update Tab" {
        n98 = Unbundle By Name(w293) -> ("Tab"=w292:T1)
        n99 = Type Cast(type=0, x=w292) -> (*(type *) &x=w290:i32)
        n100 = case shown="1" w290 {
          frame Default {
          }
          frame 1 {
            # "Report Tab.\nIf no report, produce it."
            n101 = local write "Report"("Refreshing report.\nPlease wait... " ("Report")) -> ()
          }
        }
        n102 = call <vilib>:"Add State(s) to Queue__jki_lib_state_machine.vi"("State(s) in (\"\")"=w296) -> ("States Out"=w295:string)  [unwired: 14 in]
      }
      frame "UI: Clear" {
        # "Initialize the User Interface, here.\n(this is called automatically, by the Macro: Init)"
        n103 = disable-structure shown="Default" {
          disable-tunnel: w301 -> [w307 w310]
          disable-tunnel: [w306 w310] -> w300
          frame condition #0 (active) {
            n104 = control-ref of="Tests Tree"() -> (w308:refnum<vi>)
            n105 = property on="Report" class="Str"("Text.FontName"="Courier New" ("Text.Font:Name")) -> ()  [unwired: 2 in, 2 out]
            n106 = invoke class="Tree (strict)" method="Edit Tree Items.Delete"(reference=w308, error in=w307, "Delete Children"=TRUE ("Delete Children?")) -> (error out=w306:errorcluster)  [unwired: 2 in, 4 out]
          }
          frame condition #1 {
          }
        }
        n107 = local write "Report"("") -> ()
        n108 = call <vilib>:"Add State(s) to Queue__jki_lib_state_machine.vi"("State(s) in (\"\")"=w304) -> ("States Out"=w303:string)  [unwired: 14 in]
      }
      frame "UI: Update" {
        n109 = call <vilib>:"Add State(s) to Queue__jki_lib_state_machine.vi"("State(s) in Front (\"\")"="UI: Defer Updates >> True\nUI: Clear\nUI: Update Asserts\nUI: Update Counts\nUI: Update State\nUI: Set Last Update\nUI: Defer Updates >> False", "State(s) in (\"\")"=w316) -> ("States Out"=w315:string)  [unwired: 13 in]
      }
      frame "UI: Update?" {
        n110 = Unbundle By Name(w318) -> ("Last Update"=w323:u32, "Update Delay"=w320:u32)
        n111 = Tick Count (ms)() -> (millisecond timer value=w324:u32)
        n112 = Subtract(x=w324, y=w323) -> (x-y=w322:u32)
        n113 = Greater?(x=w322, y=w320) -> (0:w319:bool)
        n114 = Select(t="UI: Update" ("State(s) in Front (\"\")"), s=w319, f="") -> (s? t:f=w321:string)
        n115 = call <vilib>:"Add State(s) to Queue__jki_lib_state_machine.vi"("State(s) in Front (\"\")"=w321, "State(s) in (\"\")"=w329) -> ("States Out"=w328:string)  [unwired: 13 in]
      }
      frame "UI: Open" {
        n116 = Unbundle By Name(w333) -> ("Interactive"=w331:bool)
        n117 = Select(t="UI: Front Panel State >> Open" ("State(s) in Front (\"\")"), s=w331, f="") -> (s? t:f=w334:string)
        n118 = call <vilib>:"Add State(s) to Queue__jki_lib_state_machine.vi"("State(s) in Front (\"\")"=w334, "State(s) in (\"\")"=w339) -> ("States Out"=w338:string)  [unwired: 13 in]
      }
      frame "UI: About" {
        n119 = disable-structure shown="Default" {
          disable-tunnel: w342 -> [w349 w351]
          disable-tunnel: [w348 w351] -> w341
          frame condition #0 (active) {
            n120 = vi-ref "About.vi"() -> (w350:refnum<vi>)
            n121 = invoke class="VI" method="Run VI"(reference=w350, error in=w349, "Wait until done"=FALSE ("Wait Until Done"), "Auto Dispose Ref"=TRUE ("Auto Dispose Reference")) -> (error out=w348:errorcluster)  [unwired: 1 in, 4 out]
          }
          frame condition #1 {
          }
        }
        n122 = call <vilib>:"Add State(s) to Queue__jki_lib_state_machine.vi"("State(s) in (\"\")"=w345) -> ("States Out"=w344:string)  [unwired: 14 in]
      }
      frame "UI: Homepage" {
        n123 = disable-structure shown="Default" {
          disable-tunnel: [w360 w361] -> w354
          disable-tunnel: w353 -> [w359 w361]
          frame condition #0 (active) {
            n124 = call-poly <vilib>:"Open URL in Default Browser.vi"("error in (no error)"=w359, "URL"="https://github.com/JKISoftware/Caraya") -> ("error out"=w360:errorcluster)  [unwired: 4 in, 1 out]
          }
          frame condition #1 {
          }
        }
        n125 = call <vilib>:"Add State(s) to Queue__jki_lib_state_machine.vi"("State(s) in (\"\")"=w357) -> ("States Out"=w356:string)  [unwired: 14 in]
      }
      frame "UI: Notify" {
        n126 = disable-structure shown="Default" {
          disable-tunnel: w364 -> [w369 w372]
          disable-tunnel: [w368 w372] -> w363
          frame condition #0 (active) {
            n127 = control-ref of="This VI"() -> (w371:refnum<vi>)
            n128 = property class="VI"(reference=w371, error in=w369, "Front Panel.IsFrontmost"=TRUE ("Front Panel Window:Is Frontmost")) -> (error out=w368:errorcluster)  [unwired: 1 out]
          }
          frame condition #1 {
          }
        }
        n129 = call <vilib>:"Add State(s) to Queue__jki_lib_state_machine.vi"("State(s) in (\"\")"=w367) -> ("States Out"=w366:string)  [unwired: 14 in]
      }
      frame "UI: Set Last Update" {
        # "Geometric progression of update refreshes.\nThe more tests there are, the longer the app\nwaits before refreshing the tree.\n\nThis is not a solid solution, but it will mitigate\nthe lagging for large number of tests in interactive mode."
        n130 = Unbundle By Name(w377) -> ("Update Delay"=w376:u32)
        n131 = Tick Count (ms)() -> (millisecond timer value=w381:u32)
        n132 = Multiply(x=2.0, y=w376) -> (x*y=w379:dbl)
        n133 = To Unsigned Long Integer(number=w379) -> (unsigned 32bit integer=w378:u32)
        n134 = Select(t=w378, s=TRUE, f=w376) -> (s? t:f=w375:u32)
        n135 = Bundle By Name(cluster=w377, "Last Update"=w381, "Update Delay"=w375) -> (w382:T8)
        n136 = call <vilib>:"Add State(s) to Queue__jki_lib_state_machine.vi"("State(s) in (\"\")"=w385) -> ("States Out"=w384:string)  [unwired: 14 in]
      }
      frame "UI: Initialize Icons" {
        # "Initialize the User Interface, here.\n(this is called automatically, by the Macro: Init)"
        n137 = disable-structure shown="Default" {
          disable-tunnel: [w394 w405] -> w388
          disable-tunnel: w387 -> [w393 w405]
          frame condition #0 (active) {
            w392 = cluster{"Image":T12, "Index":T13}[] [{"Image"={"image type"=0, "image depth"=32, "image"=array[1024 elements], "mask"=[255, 255, 255, 255, 255, 255, 255, 255, 255, 255, 255, 255, 255, 255, 255, 255, 255, 255, 255, 255, 255, 255, 255, 255, 255, 255, 255, 255, 255, 255, 255, 255], "colors"=[], "Rectangle"={"left"=0, "top"=0, "right"=16, "bottom"=16}}, "Index"=enum."Unknown"}, {"Image"={"image type"=0, "image depth"=32, "image"=array[1024 elements], "mask"=[255, 255, 255, 255, 255, 255, 255, 255, 255, 255, 255, 255, 255, 255, 255, 255, 255, 255, 255, 255, 255, 255, 255, 255, 255, 255, 255, 255, 255, 255, 255, 255], "colors"=[], "Rectangle"={"left"=0, "top"=0, "right"=16, "bottom"=16}}, "Index"=enum."Fail"}, {"Image"={"image type"=0, "image depth"=32, "image"=array[1024 elements], "mask"=[255, 255, 255, 255, 255, 255, 255, 255, 255, 255, 255, 255, 255, 255, 255, 255, 255, 255, 255, 255, 255, 255, 255, 255, 255, 255, 255, 255, 255, 255, 255, 255], "colors"=[], "Rectangle"={"left"=0, "top"=0, "right"=16, "bottom"=16}}, "Index"=enum."Pass"}, {"Image"={"image type"=0, "image depth"=32, "image"=array[1024 elements], "mask"=[255, 255, 255, 255, 255, 255, 255, 255, 255, 255, 255, 255, 255, 255, 255, 255, 255, 255, 255, 255, 255, 255, 255, 255, 255, 255, 255, 255, 255, 255, 255, 255], "colors"=[], "Rectangle"={"left"=0, "top"=0, "right"=16, "bottom"=16}}, "Index"=enum."Skip"}, {"Image"={"image type"=0, "image depth"=32, "image"=array[1024 elements], "mask"=[255, 255, 255, 255, 255, 255, 255, 255, 255, 255, 255, 255, 255, 255, 255, 255, 255, 255, 255, 255, 255, 255, 255, 255, 255, 255, 255, 255, 255, 255, 255, 255], "colors"=[], "Rectangle"={"left"=0, "top"=0, "right"=16, "bottom"=16}}, "Index"=enum."Error"}, {"Image"={"image type"=0, "image depth"=32, "image"=array[1024 elements], "mask"=[255, 255, 255, 255, 255, 255, 255, 255, 255, 255, 255, 255, 255, 255, 255, 255, 255, 255, 255, 255, 255, 255, 255, 255, 255, 255, 255, 255, 255, 255, 255, 255], "colors"=[], "Rectangle"={"left"=0, "top"=0, "right"=16, "bottom"=16}}, "Index"=enum."Fail Node"}, {"Image"={"image type"=0, "image depth"=32, "image"=array[1024 elements], "mask"=[255, 255, 255, 255, 255, 255, 255, 255, 255, 255, 255, 255, 255, 255, 255, 255, 255, 255, 255, 255, 255, 255, 255, 255, 255, 255, 255, 255, 255, 255, 255, 255], "colors"=[], "Rectangle"={"left"=0, "top"=0, "right"=16, "bottom"=16}}, "Index"=enum."Pass Node"}]  # Tree Icons
            n138 = control-ref of="Tests Tree"() -> (w395:refnum<vi>)
            n139 = property class="Tree (strict)"(reference=w395, error in=w393, "SymsVis"=TRUE ("Visible Items:Symbols Visible")) -> (reference out=w397:refnum<vi>, error out=w396:errorcluster)
            n140 = for {
              tunnel: w397 -> [w404]
              tunnel: w392 -> [w403] mode=indexing
              shift-right: [w400] -> w394
              shift-left: w396 -> [w401]
              n141 = Unbundle By Name(w403) -> ("Index"=w399:T13, "Image"=w402:T12)
              n142 = invoke class="Tree (strict)" method="Custom Item Symbols.Set Symbol"(reference=w404, error in=w401, "index"=w399, "image"=w402) -> (error out=w400:errorcluster)  [unwired: 1 in, 4 out]
            }
          }
          frame condition #1 {
          }
        }
        n143 = call <vilib>:"Add State(s) to Queue__jki_lib_state_machine.vi"("State(s) in (\"\")"=w391) -> ("States Out"=w390:string)  [unwired: 14 in]
      }
      frame "UI: Update Asserts" {
        # "Initialize the User Interface, here.\n(this is called automatically, by the Macro: Init)"
        n144 = disable-structure shown="Default" {
          disable-tunnel: w409 -> [w421 _]
          disable-tunnel: [w423 w456] -> w408
          disable-tunnel: w407 -> [w422 w456]
          frame condition #0 (active) {
            n145 = control-ref of="Tests Tree"() -> (w418:refnum<vi>)
            n146 = Unbundle By Name(w421) -> ("Storage"=w420:refnum<class "Test Event Storage.lvclass">)
            n147 = Unbundle By Name(w421) -> ("Hide Passed Tests"=w417:bool)
            n148 = call-dynamic "Get All Test Registrations.vi"("error in (no error)"=w422, "Test Event Storage in"=w420) -> ("error out"=w414:errorcluster, "Test Registrations"=w413:T3[], "Test IDs"=w415:string[], "Test Event Storage out"=w419:refnum<class "Test Event Storage.lvclass">, "Test Parent IDs"=w416:string[])  [unwired: 5 in]
            n149 = Empty Array?(array=w413) -> (empty?=w412:bool)
            n150 = case shown="False" w412 {
              tunnel: [w436 w454] -> w423
              tunnel: w419 -> [w435 _]
              tunnel: w418 -> [w434 w455]
              tunnel: w417 -> [w432 _]
              tunnel: w416 -> [w431 _]
              tunnel: w415 -> [w430 _]
              tunnel: w414 -> [w428 _]
              tunnel: w413 -> [w425 _]
              frame False {
                # "TODO: Filter orphaned tests (no asserts)\n-- Use Defined Test flag??"
                n151 = for {
                  tunnel: w430 -> [w437] mode=indexing
                  tunnel: w425 -> [w440] mode=indexing
                  shift-right: [w441] -> w427
                  shift-left: w428 -> [w442]
                  shift-right: [w443] -> w433
                  shift-left: w434 -> [w444]
                  tunnel: w431 -> [w439] mode=indexing
                  tunnel: w432 -> [w438]
                  n152 = call "Add Node To Tree.vi"("Hide Passes"=w438, "Parent Key"=w439, "error in (no error)"=w442, "Test Node"=w440, "Key"=w437, "tree refnum"=w444) -> ("error out"=w441:errorcluster, "dup tree refnum"=w443:refnum<vi>)  [unwired: 4 in]
                }
                n153 = call-dynamic "Get All Test Events.vi"("error in (no error)"=w427, "Test Event Storage in"=w435) -> ("error out"=w426:errorcluster, "Test IDs"=w429:string[], "Assertions"=w424:T14[])  [unwired: 6 in, 1 out]
                n154 = for {
                  tunnel: w429 -> [w449] mode=indexing
                  shift-right: [w446] -> w436
                  shift-left: w426 -> [w448]
                  shift-right: [w447] -> _
                  shift-left: w433 -> [w450]
                  tunnel: w424 -> [w445] mode=indexing
                  n155 = call "Add Test Event To Tree.vi"("error in (no error)"=w448, "Assert Event Data"=w445, "Parent Key"=w449, "tree refnum"=w450) -> ("error out"=w446:errorcluster, "dup tree refnum"=w447:refnum<vi>)  [unwired: 6 in]
                }
              }
              frame True {
                n156 = Bundle By Name(cluster=T3 {"Test Registration"={"Name"="", "Call Chain"=[], "Time Stamp"=timestamp(0 s since 1904-01-01), "Test ID"="", "Caller ID"=""}, "Defined"=FALSE, "Passed"=FALSE, "properties"=variant} ("Test Node"), "Test Registration.Name"="No tests found. (Ensure all your project’s tests are saved to disk before calling Run Tests)" ("Key")) -> (w453:T3)
                n157 = call "Add Node To Tree.vi"("Test Node"=w453, "tree refnum"=w455) -> ("error out"=w454:errorcluster)  [unwired: 8 in, 1 out]
              }
            }
          }
          frame condition #1 {
          }
        }
        n158 = call <vilib>:"Add State(s) to Queue__jki_lib_state_machine.vi"("State(s) in (\"\")"=w411) -> ("States Out"=w410:string)  [unwired: 14 in]
      }
      frame "UI: Update Counts" {
        n159 = Unbundle By Name(w458) -> ("Storage"=w460:refnum<class "Test Event Storage.lvclass">)
        n160 = disable-structure shown="TARGET_TYPE!=RT, Default" {
          disable-tunnel: w461 -> [w480 w500]
          disable-tunnel: w460 -> [w479 _]
          disable-tunnel: [w465 w500] -> w459
          frame condition #0 (active) {
            w475 = T7[] [enum."Unknown", enum."Skip", enum."Pass", enum."Fail", enum."Error"] items=["Empty", "Unknown", "Fail", "Pass", "Skip", "Error"]
            w473 = string[] ["Unknowns", "Skipped", "Passed", "Failed", "Errors"]  # Plural
            w474 = string[] ["Unknown", "Skipped", "Passed", "Failed", "Error"]  # Singular
            n161 = call-dynamic "Get All Test Events.vi"("error in (no error)"=w480, "Test Event Storage in"=w479) -> ("error out"=w478:errorcluster, "Assertions"=w464:T14[])  [unwired: 6 in, 2 out]
            n162 = for {
              shift-right: [w498] -> w466
              shift-left: w478 -> [w497]
              tunnel: [w499] -> w477 mode=indexing
              tunnel: w464 -> [w496] mode=indexing
              n163 = call "Test State.vi"("error in (no error)"=w497, "Assert Event Data"=w496) -> ("error out"=w498:errorcluster, "Test State"=w499:T7)  [unwired: 8 in]
            }
            n164 = Sort 1D Array(array=w477) -> (sorted array=w476:T7[])
            n165 = control-ref of="Unknown String"() -> (w472:refnum<vi>)
            n166 = control-ref of="Skip String"() -> (w471:refnum<vi>)
            n167 = control-ref of="Pass String"() -> (w470:refnum<vi>)
            n168 = control-ref of="Fail String"() -> (w469:refnum<vi>)
            n169 = control-ref of="Error String"() -> (w468:refnum<vi>)
            n170 = Build Array(w472, w471, w470, w469, w468) -> (w467:refnum<vi>[])
            n171 = for {
              tunnel: w476 -> [w485]
              tunnel: w475 -> [w484] mode=indexing
              tunnel: w474 -> [w493] mode=indexing
              tunnel: w473 -> [w492] mode=indexing
              tunnel: w467 -> [w489] mode=indexing
              shift-right: [w487] -> w465
              shift-left: w466 -> [w486]
              n172 = Equal?(x=w485, y=w484) -> (x = y?=w483:bool[])
              n173 = Boolean To (0,1)(Boolean=w483) -> (0, 1=w482:i16[])
              n174 = Add Array Elements(numeric array=w482) -> (sum=w481:i16)
              n175 = Equal?(x=i16 1, y=w481) -> (x = y?=w494:bool)
              n176 = Select(t=w493, s=w494, f=w492) -> (s? t:f=w490:string)
              n177 = Format Into String(format string="%d %s", w481, w490) -> (resulting string=w488:string)  [unwired: 2 in, 1 out]
              n178 = property class="Str"(reference=w489, error in=w486, "Value"=w488) -> (error out=w487:errorcluster)  [unwired: 1 out]
            }
          }
          frame condition #1 {
          }
        }
        n179 = call <vilib>:"Add State(s) to Queue__jki_lib_state_machine.vi"("State(s) in (\"\")"=w463) -> ("States Out"=w462:string)  [unwired: 14 in]
      }
      frame "UI: Update State" {
        # "Initialize the User Interface, here.\n(this is called automatically, by the Macro: Init)"
        n180 = disable-structure shown="Default" {
          disable-tunnel: w502 -> [w518 _]
          frame condition #0 (active) {
            n181 = Unbundle By Name(w518) -> ("Final State"=w517:T7, "Hide Passed Tests"=w513:bool)
            n182 = case shown="\"Fail\", \"Error\"" w517 {
              tunnel: [w522 w525 TRUE] -> w514
              tunnel: [w522 TRUE w531] -> w516
              tunnel: [TRUE w525 w531] -> w515
              tunnel: [T5."Page Enabled" ("Page Enabled State") T5."Page Enabled" ("Page Enabled State") T5."Page Disabled & Grayed" ("Page Enabled State")] -> w506
              tunnel: [w520 w524 w528] -> w510
              frame "Pass", "Skip" {
                w522 = FALSE
                n183 = local read "Tab"() -> (w520:T1)
              }
              frame "Fail", "Error" {
                w525 = FALSE
                n184 = local read "Tab"() -> (w524:T1)
              }
              frame "Unknown", Default {
                w531 = FALSE
                n185 = local read "Tab"() -> (w529:T1)
                n186 = Type Cast(type=w529, x=0) -> (*(type *) &x=w528:T1)
              }
            }
            n187 = property on="Tab" class="TabCtl (strict)"() -> ("Pages"=w509:refnum<vi>[])  [unwired: 2 in, 2 out]
            n188 = Index Array(array=w509, index=1) -> (element=w507:refnum<vi>)
            n189 = local write "Hide Passed Tests Checkbox"(w513) -> ()
            n190 = property on="Unknow" class="Bool (strict)"("Visible"=w514) -> ()  [unwired: 2 in, 2 out]
            n191 = property on="Fail" class="Bool (strict)"("Visible"=w516) -> ()  [unwired: 2 in, 2 out]
            n192 = property on="Pass" class="Bool (strict)"("Visible"=w515) -> ()  [unwired: 2 in, 2 out]
            n193 = local write "Tab"(w510) -> ()
            n194 = property on="Property Node" class="Page"(reference=w507, "PageEnb"=w506) -> ()  [unwired: 1 in, 2 out]
            n195 = Equal To 0?(x=w510) -> (x = 0?=w511:bool)
            n196 = Not(x=w511) -> (.not. x?=w512:bool)
            n197 = property on="Report" class="Str"("Visible"=w512) -> ()  [unwired: 2 in, 2 out]
            n198 = property on="Tests Tree" class="Tree (strict)"("Visible"=w511) -> ()  [unwired: 2 in, 2 out]
          }
          frame condition #1 {
          }
        }
        n199 = call <vilib>:"Add State(s) to Queue__jki_lib_state_machine.vi"("State(s) in (\"\")"=w505) -> ("States Out"=w504:string)  [unwired: 14 in]
      }
      frame "UI: Cursor Set" {
        # "Argument"
        # "Set and Unset Cursor Busy.\n(Usage: \"UI: Cursor Set >> Busy|Idle\")"
        n200 = disable-structure shown="Default" {
          disable-tunnel: w536 -> [w542 w547]
          disable-tunnel: [w541 w547] -> w535
          disable-tunnel: w534 -> [w540 _]
          frame condition #0 (active) {
            n201 = case shown="\"Idle\", Default" w540 {
              tunnel: w542 -> [w544 w546]
              tunnel: [w543 w545] -> w541
              frame "Idle", Default {
                n202 = call <vilib>:"Unset Busy.vi"("error in (no error)"=w544) -> ("error out"=w543:errorcluster)  [unwired: 10 in]
              }
              frame "Busy" {
                n203 = call <vilib>:"Set Busy.vi"("error in (no error)"=w546) -> ("error out"=w545:errorcluster)  [unwired: 9 in, 1 out]
              }
            }
          }
          frame condition #1 {
          }
        }
        n204 = call <vilib>:"Add State(s) to Queue__jki_lib_state_machine.vi"("State(s) in (\"\")"=w539) -> ("States Out"=w538:string)  [unwired: 14 in]
      }
      frame "UI: Defer Updates" {
        # "Argument"
        n205 = Unbundle By Name(w551) -> ("Core.Current VI Reference"=w550:refnum<vi>)
        n206 = case shown="\"True\"" w553 {
          tunnel: [_ TRUE] -> w554
          frame "False", Default {
          }
          frame "True" {
          }
        }
        n207 = disable-structure shown="Default" {
          disable-tunnel: w554 -> [w563 _]
          disable-tunnel: w549 -> [w560 w566]
          disable-tunnel: [w559 w566] -> w552
          disable-tunnel: w550 -> [w557 _]
          frame condition #0 (active) {
            n208 = property class="VI"(reference=w557) -> (error out=w564:errorcluster, "Panel"=w565:refnum<vi>)  [unwired: 1 in, 1 out]
            n209 = property class="Pnl"(reference=w565, error in=w564, "DeferPanUpdts"=w563) -> (reference out=w561:refnum<vi>, error out=w562:errorcluster)
            n210 = Close Reference(reference=w561, error in (no error)=w562) -> (error out=w558:errorcluster)
            n211 = Merge Errors(w560, w558) -> (w559:errorcluster)
          }
          frame condition #1 {
          }
        }
        n212 = call <vilib>:"Add State(s) to Queue__jki_lib_state_machine.vi"("State(s) in (\"\")"=w556) -> ("States Out"=w555:string)  [unwired: 14 in]
      }
      frame "UI: Front Panel State" {
        # "Set Front Panel Open or Closed\n(Usage: \"UI: Front Panel State >> Open|Close\")"
        n213 = disable-structure shown="Default" {
          disable-tunnel: w572 -> [w579 w602]
          disable-tunnel: [w578 w602] -> w571
          disable-tunnel: w570 -> [w577 _]
          disable-tunnel: w569 -> [w575 _]
          frame condition #0 (active) {
            # "Argument"
            n214 = Unbundle By Name(w577) -> ("Core.Current VI Reference"=w576:refnum<vi>)
            n215 = case shown="\"Close\"" w575 {
              tunnel: w579 -> [w583 w596]
              tunnel: [w585 w597] -> w578
              tunnel: w576 -> [w584 w594]
              frame "Open", Default {
                n216 = property class="VI"(reference=w584, error in=w583) -> (reference out=w581:refnum<vi>, error out=w582:errorcluster, "Front Panel.Open"=w580:bool)
                n217 = case shown="False" w580 {
                  tunnel: [w588 w591] -> w585
                  tunnel: w582 -> [w587 w591]
                  tunnel: w581 -> [w586 _]
                  frame False {
                    n218 = invoke class="VI" method="FP.Open"(reference=w586, error in=w587, "Activate"=TRUE, "State"=T6."Standard") -> (error out=w588:errorcluster)  [unwired: 1 in, 4 out]
                  }
                  frame True {
                  }
                }
              }
              frame "Close" {
                n219 = property class="VI"(reference=w594, error in=w596) -> (reference out=w593:refnum<vi>, error out=w595:errorcluster, "Front Panel.Open"=w592:bool)
                n220 = case shown="True" w592 {
                  tunnel: [w598 w601] -> w597
                  tunnel: w595 -> [w598 w600]
                  tunnel: w593 -> [_ w599]
                  frame False {
                  }
                  frame True {
                    n221 = invoke class="VI" method="FP.Close"(reference=w599, error in=w600) -> (error out=w601:errorcluster)  [unwired: 1 in, 2 out]
                  }
                }
              }
            }
          }
          frame condition #1 {
          }
        }
        n222 = call <vilib>:"Add State(s) to Queue__jki_lib_state_machine.vi"("State(s) in (\"\")"=w574) -> ("States Out"=w573:string)  [unwired: 14 in]
      }
      frame "---------- Macro ----------" {
        # "Do not put any code in this frame.\n(It is a separator no-op. You can make a copy of this frame to create a new Macro frame)"
        n223 = call <vilib>:"Add State(s) to Queue__jki_lib_state_machine.vi"("State(s) in (\"\")"=w607) -> ("States Out"=w606:string)  [unwired: 14 in]
      }
      frame "Macro: Initialize" {
        # "Initialization Macro\n(This is called once, when the VI starts)"
        n224 = call <vilib>:"Add State(s) to Queue__jki_lib_state_machine.vi"("State(s) in Front (\"\")"="Data: Initialize\nInitialize Core Data\nEvent: Register\nUI: Initialize\nUI: Open", "State(s) in (\"\")"=w613) -> ("States Out"=w612:string)  [unwired: 13 in]
      }
      frame "Macro: Complete" {
        n225 = call <vilib>:"Add State(s) to Queue__jki_lib_state_machine.vi"("State(s) in Front (\"\")"="Test: Complete\nTest: Publish Test Result\nTest: Export Report\nTest: Notify\nTest: Exit?\nUI: Notify\nUI: Update", "State(s) in (\"\")"=w619) -> ("States Out"=w618:string)  [unwired: 13 in]
      }
      frame "Macro: Rerun" {
        n226 = call <vilib>:"Add State(s) to Queue__jki_lib_state_machine.vi"("State(s) in Front (\"\")"="Test: Rerun", "State(s) in (\"\")"=w625) -> ("States Out"=w624:string)  [unwired: 13 in]
      }
      frame "Macro: Export" {
        n227 = call <vilib>:"Add State(s) to Queue__jki_lib_state_machine.vi"("State(s) in Front (\"\")"="Test: Export?", "State(s) in (\"\")"=w631) -> ("States Out"=w630:string)  [unwired: 13 in]
      }
      frame "Macro: Export JUnit" {
        n228 = call <vilib>:"Add State(s) to Queue__jki_lib_state_machine.vi"("State(s) in Front (\"\")"="Test: Export? >> JUnit", "State(s) in (\"\")"=w637) -> ("States Out"=w636:string)  [unwired: 13 in]
      }
      frame "Macro: Exit" {
        # "JK 2016-08-26 - Moved \"UI: Clear\" into Macro Exit, since it seemed to be called right before \"Macro: Exit\" nearly everywhere."
        # "Exit Macro\n(This is called once, when the VI exits)"
        n229 = Unbundle By Name(w646) -> ("Core.Close Panel on Exit?"=w645:bool)
        n230 = Select(t="UI: Front Panel State >> Close", s=w645, f="") -> (s? t:f=w642:string)
        n231 = call <vilib>:"Add State(s) to Queue__jki_lib_state_machine.vi"("State(s) in Front (\"\")"="UI: Clear" ("State(s) in Front (\"\")"), "State(s) in (\"\")"=w642, "State(s) at Back (\"\")"="Data: Cleanup\nExit") -> ("States Out"=w640:string)  [unwired: 12 in]
        n232 = call <vilib>:"Add State(s) to Queue__jki_lib_state_machine.vi"("State(s) in Front (\"\")"=w640, "State(s) in (\"\")"=w649) -> ("States Out"=w648:string)  [unwired: 13 in]
      }
      frame "---------- Assert ----------" {
        # "Template Separator\n(You can make a copy of, or modify, this frame)"
        n233 = call <vilib>:"Add State(s) to Queue__jki_lib_state_machine.vi"("State(s) in (\"\")"=w654) -> ("States Out"=w653:string)  [unwired: 14 in]
      }
      frame "Assert: Register" {
        n234 = Unbundle By Name(w655) -> ("Message"=w662:refnum<class "TestManagerMsg.lvclass">)
        n235 = To More Specific Class(target class=refnum<class "TestManagerMsg.Assertion.lvclass"> refnum ("Message.Assertion"), reference=w662, error in=w660) -> (specific class reference=w657:refnum<class "TestManagerMsg.Assertion.lvclass">, error out=w656:errorcluster)
        n236 = in-place {
          in-place-border: [w672] -> w663
          in-place-border: w656 -> [w669]
          in-place-border: w657 -> [w667]
          n237 = in-place-cluster #1(w655) -> ("State"=w676:T7, "Storage"=w671:refnum<class "Test Event Storage.lvclass">)
          n238 = call "To Test Event.vi"("TestManagerMsg.Assertion in"=w667) -> ("Assert Event Data"=w668:T14)  [unwired: 10 in]
          n239 = call "Resolve New State.vi"("error in"=w669, "Assert Event Data"=w668, "Current State"=w676) -> ("error out"=w673:errorcluster, "New State"=w675:T7)  [unwired: 7 in]
          n240 = call-dynamic "New-Update Assertion.vi"("error in (no error)"=w669, "Assertion"=w667, "Test Event Storage in"=w671) -> ("error out"=w674:errorcluster, "Test Event Storage out"=w670:refnum<class "Test Event Storage.lvclass">)  [unwired: 6 in, 1 out]
          n241 = Merge Errors(w673, w674) -> (w672:errorcluster)
          n242 = in-place-cluster #1("State"=w675, "Storage"=w670) -> (w664:T8)
        }
        n243 = call "Send Assertion Event.vi"("error in (no error)"=w656, "Message"=w657, "Basic Test Manager in"=w658) -> ()  [unwired: 7 in, 2 out]
        n244 = call <vilib>:"Add State(s) to Queue__jki_lib_state_machine.vi"("State(s) in (\"\")"=w666) -> ("States Out"=w665:string)  [unwired: 14 in]
      }
      frame "Assert: Update Explanation" {
        n245 = Unbundle By Name(w683) -> ("Message"=w686:refnum<class "TestManagerMsg.lvclass">)
        n246 = To More Specific Class(target class=refnum<class "TestManagerMsg.Verbose.lvclass"> refnum ("Caraya.lvlib:TestManagerMsg.Verbose.lvclass"), reference=w686, error in=w684) -> (specific class reference=w680:refnum<class "TestManagerMsg.Verbose.lvclass">, error out=w679:errorcluster)
        n247 = case shown="No Error" w679 {
          selector: w679 -> [w689 w700]
          tunnel: [w694 w701] -> w677
          tunnel: [w693 w700] -> w678
          tunnel: w683 -> [w692 w701]
          tunnel: w681 -> [w691 _]
          tunnel: w680 -> [w690 _]
          frame No Error {
            n248 = in-place {
              in-place-border: w689 -> [w698]
              in-place-border: [w699] -> w693
              in-place-border: w690 -> [w695]
              n249 = in-place-cluster #2(w692) -> ("Storage"=w697:refnum<class "Test Event Storage.lvclass">)
              n250 = call-dynamic "Update Verbose Explanation.vi"("error in (no error)"=w698, "Verbose"=w695, "Test Event Storage in"=w697) -> ("error out"=w699:errorcluster, "Test Event Storage out"=w696:refnum<class "Test Event Storage.lvclass">)  [unwired: 7 in]
              n251 = in-place-cluster #2("Storage"=w696) -> (w694:T8)
            }
            n252 = call "Send Assertion Update.vi"("Message"=w690, "Basic Test Manager in"=w691) -> ()  [unwired: 8 in, 2 out]
          }
          frame Error {
          }
        }
        n253 = call <vilib>:"Add State(s) to Queue__jki_lib_state_machine.vi"("State(s) in (\"\")"=w687) -> ("States Out"=w688:string)  [unwired: 14 in]
      }
      frame "Assert: Add Key-Value Pair" {
        n254 = Unbundle By Name(w709) -> ("Message"=w710:refnum<class "TestManagerMsg.lvclass">)
        n255 = To More Specific Class(target class=refnum<class "TestManagerMsg.KVP.lvclass"> refnum ("Caraya.lvlib:TestManagerMsg.KVP.lvclass"), reference=w710, error in=w704) -> (specific class reference=w708:refnum<class "TestManagerMsg.KVP.lvclass">, error out=w706:errorcluster)
        n256 = case shown="No Error" w706 {
          selector: w706 -> [_ w724]
          tunnel: [w719 w725] -> w713
          tunnel: [w718 w724] -> w703
          tunnel: w711 -> [w716 _]
          tunnel: w709 -> [w717 w725]
          tunnel: w708 -> [w715 _]
          frame No Error {
            n257 = in-place {
              in-place-border: [w723] -> w718
              in-place-border: w715 -> [w720]
              n258 = in-place-cluster #3(w717) -> ("Storage"=w722:refnum<class "Test Event Storage.lvclass">)
              n259 = call-dynamic "Update Test-Assertion KVP.vi"("KVP"=w720, "Test Event Storage in"=w722) -> ("error out"=w723:errorcluster, "Test Event Storage out"=w721:refnum<class "Test Event Storage.lvclass">)  [unwired: 8 in]
              n260 = in-place-cluster #3("Storage"=w721) -> (w719:T8)
            }
            n261 = call "Send Assertion Update.vi"("Message"=w715, "Basic Test Manager in"=w716) -> ()  [unwired: 8 in, 2 out]
          }
          frame Error {
          }
        }
        n262 = Merge Errors(w704, w703) -> (w702:errorcluster)
        n263 = call <vilib>:"Add State(s) to Queue__jki_lib_state_machine.vi"("State(s) in (\"\")"=w712) -> ("States Out"=w714:string)  [unwired: 14 in]
      }
      frame "Assert: Add Measurement" {
        n264 = Unbundle By Name(w731) -> ("Message"=w732:refnum<class "TestManagerMsg.lvclass">)
        n265 = To More Specific Class(target class=refnum<class "TestManagerMsg.Measurement.lvclass"> refnum ("Caraya.lvlib:TestManagerMsg.Measurement.lvclass"), reference=w732, error in=w728) -> (specific class reference=w730:refnum<class "TestManagerMsg.Measurement.lvclass">, error out=w729:errorcluster)
        n266 = case shown="No Error" w729 {
          tunnel: [w743 w749] -> w736
          tunnel: [w742 w750] -> w735
          tunnel: w733 -> [w739 _]
          tunnel: w731 -> [w741 w749]
          tunnel: w730 -> [w738 _]
          tunnel: w728 -> [w740 w750]
          frame No Error {
            n267 = in-place {
              in-place-border: w740 -> [w745]
              in-place-border: [w744] -> w742
              in-place-border: w738 -> [w746]
              n268 = in-place-cluster #4(w741) -> ("Storage"=w748:refnum<class "Test Event Storage.lvclass">)
              n269 = call-dynamic "Update Test-Assertion Measurement.vi"("error in (no error)"=w745, "Measurement"=w746, "Test Event Storage in"=w748) -> ("error out"=w744:errorcluster, "Test Event Storage out"=w747:refnum<class "Test Event Storage.lvclass">)  [unwired: 7 in]
              n270 = in-place-cluster #4("Storage"=w747) -> (w743:T8)
            }
            n271 = call "Send Assertion Update.vi"("Message"=w738, "Basic Test Manager in"=w739) -> ()  [unwired: 8 in, 2 out]
          }
          frame Error {
          }
        }
        n272 = call <vilib>:"Add State(s) to Queue__jki_lib_state_machine.vi"("State(s) in (\"\")"=w734) -> ("States Out"=w737:string)  [unwired: 14 in]
      }
      frame "---------- TestMngr ----------" {
        # "Template Separator\n(You can make a copy of, or modify, this frame)"
        n273 = call <vilib>:"Add State(s) to Queue__jki_lib_state_machine.vi"("State(s) in (\"\")"=w755) -> ("States Out"=w754:string)  [unwired: 14 in]
      }
      frame "TestMngr: Check Running" {
        # "Trigger once when tests stop running"
        n274 = call "Register Check Running.vi"("error in (no error)"=w768, "Check Running (F)"=TRUE) -> ("error out"=w767:errorcluster, "Running?"=w759:bool)  [unwired: 8 in]
        n275 = Unbundle By Name(w763) -> ("Complete"=w761:bool, "Running"=w758:bool)
        n276 = Equal?(x=w758, y=w759) -> (x = y?=w757:bool)
        n277 = Or(x=w757, y=w759) -> (x .or. y?=w762:bool)
        n278 = Or(x=w761, y=w762) -> (x .or. y?=w760:bool)
        n279 = Select(t="", s=w760, f="Macro: Complete") -> (s? t:f=w764:string)
        n280 = call <vilib>:"Add State(s) to Queue__jki_lib_state_machine.vi"("State(s) in Front (\"\")"=w764, "State(s) in (\"\")"=w771) -> ("States Out"=w770:string)  [unwired: 13 in]
      }
      frame "---------- Test ----------" {
        # "Template Separator\n(You can make a copy of, or modify, this frame)"
        n281 = call <vilib>:"Add State(s) to Queue__jki_lib_state_machine.vi"("State(s) in (\"\")"=w776) -> ("States Out"=w775:string)  [unwired: 14 in]
      }
      frame "Test: Register" {
        n282 = Unbundle By Name(w790) -> ("Message"=w786:refnum<class "TestManagerMsg.lvclass">, "Start Time"=w779:timestamp)
        n283 = To More Specific Class(target class=refnum<class "TestManagerMsg.Test.lvclass"> refnum ("Caraya.lvlib:TestManagerMsg.Test.lvclass"), reference=w786) -> (specific class reference=w783:refnum<class "TestManagerMsg.Test.lvclass">)  [unwired: 1 in, 1 out]
        n284 = Not Equal?(x=w779, y=timestamp(0 s since 1904-01-01) ("Start Time")) -> (x != y?=w780:bool)
        n285 = Get Date/Time In Seconds() -> (seconds since 1Jan1904=w778:timestamp)
        n286 = Select(t=w779, s=w780, f=w778) -> (s? t:f=w777:timestamp)
        n287 = call "Send Test Event.vi"("Message"=w783, "Basic Test Manager in"=w784) -> ("error out"=w782:errorcluster)  [unwired: 8 in, 1 out]
        n288 = Unbundle By Name(w790) -> ("Storage"=w788:refnum<class "Test Event Storage.lvclass">)
        n289 = call-dynamic "New-Update Test.vi"("Test"=w783, "Test Event Storage in"=w788) -> ("error out"=w792:errorcluster, "Test Event Storage out"=w789:refnum<class "Test Event Storage.lvclass">)  [unwired: 7 in, 1 out]
        n290 = Bundle By Name(cluster=w790, "Storage"=w789, "Start Time"=w777) -> (w791:T8)
        n291 = Merge Errors(w793, w792, w782) -> (w794:errorcluster)
        n292 = call <vilib>:"Add State(s) to Queue__jki_lib_state_machine.vi"("State(s) in (\"\")"=w796) -> ("States Out"=w795:string)  [unwired: 14 in]
      }
      frame "Test: Rerun" {
        n293 = Unbundle By Name(w805) -> ("Storage"=w804:refnum<class "Test Event Storage.lvclass">)
        n294 = call "Rerun Tests.vi"("error in (no error)"=w803, "Storage"=w804) -> ("error out"=w802:errorcluster, "Called Run Tests in Active Project"=w801:bool)  [unwired: 8 in]
        n295 = Select(t="Macro: Exit" ("State(s) in Front (\"\")"), s=w801, f="") -> (s? t:f=w799:string)
        n296 = call <vilib>:"Add State(s) to Queue__jki_lib_state_machine.vi"("State(s) in Front (\"\")"=w799, "State(s) in (\"\")"=w807) -> ("States Out"=w806:string)  [unwired: 13 in]
      }
      frame "Test: Open" {
        n297 = disable-structure shown="Default" {
          disable-tunnel: w813 -> [w826 w843]
          disable-tunnel: w812 -> [w824 _]
          disable-tunnel: [w820 w843] -> w811
          disable-tunnel: w810 -> [w817 _]
          frame condition #0 (active) {
            n298 = Unbundle By Name(w817) -> ("Argument"=w828:variant)
            n299 = property on="Tests Tree" class="Tree (strict)"() -> ("Cell String"=w816:string, "Child-Only?"=w821:bool, "Active Item Tag"=w815:string)  [unwired: 2 in, 2 out]
            n300 = Unbundle By Name(w817) -> ("Storage"=w818:refnum<class "Test Event Storage.lvclass">)
            n301 = Variant To Data(error in=w826, type="", Variant=w828) -> (data=w822:string, error out=w827:errorcluster)
            n302 = case shown="True" w821 {
              tunnel: w827 -> [w829 w839]
              tunnel: w822 -> [w834 _]
              tunnel: [w831 w835] -> w823
              tunnel: [w830 w838] -> w819
              tunnel: w818 -> [w832 w842]
              tunnel: w815 -> [_ w841]
              frame False {
                n303 = call "Get Test Registration by Key.vi"("error in (no error)"=w829, "Key"=w834, "Test Event Storage in"=w832) -> ("error out"=w830:errorcluster, "Test Node"=w833:T15)  [unwired: 5 in, 2 out]
                n304 = Unbundle By Name(w833) -> ("Test Registration.Call Chain"=w831:string[])
              }
              frame True {
                n305 = invoke on="Tests Tree" class="Tree (strict)" method="Navigate Tree.Get Parent"("tag"=w841) -> ("Navigate Tree:Get Parent"=w840:string)  [unwired: 3 in, 3 out]
                n306 = call "Get Tests Events by Key.vi"("error in (no error)"=w839, "Key (Test ID)"=w840, "Test Event Storage in"=w842) -> ("error out"=w838:errorcluster, "Assertions"=w837:T14[])  [unwired: 6 in, 1 out]
                n307 = Index Array(array=w837) -> (element=w836:T14)  [unwired: 1 in]
                n308 = Unbundle By Name(w836) -> ("call-chain"=w835:string[])
              }
            }
            n309 = call "Open Block Diagram.vi"("error in (no error)"=w819, "Assertion Label"=w816, "Call Chain"=w823, "Basic Test Manager in"=w824) -> ("error out"=w820:errorcluster)  [unwired: 6 in, 1 out]
          }
          frame condition #1 {
          }
        }
        n310 = call <vilib>:"Add State(s) to Queue__jki_lib_state_machine.vi"("State(s) in (\"\")"=w809) -> ("States Out"=w814:string)  [unwired: 14 in]
      }
      frame "Test: Notify" {
        n311 = Unbundle By Name(w849) -> ("State"=w847:T7, "Storage"=w853:refnum<class "Test Event Storage.lvclass">, "final error"=w854:errorcluster)
        n312 = Unbundle By Name(w849) -> ("Message"=w848:refnum<class "TestManagerMsg.lvclass">)
        n313 = To More Specific Class(target class=refnum<class "TestManagerMsg.CompleteSuite.lvclass"> refnum ("Caraya.lvlib:TestManagerMsg.CompleteSuite.lvclass"), reference=w848, error in=w846) -> (specific class reference=w850:refnum<class "TestManagerMsg.CompleteSuite.lvclass">, error out=w851:errorcluster)
        n314 = case shown="No Error" w851 {
          tunnel: w847 -> [w865 _]
          tunnel: w854 -> [w863 _]
          tunnel: w853 -> [w862 _]
          tunnel: w850 -> [w861 _]
          frame No Error {
            # "[Fix: 4]"
            # "Ignore Error. The lifetime\nof notifier is managed in\nanother thread"
            n315 = call "Read Notifier.vi"("TestManagerMsg.CompleteSuite in"=w861) -> ("notifier"=w860:refnum<notifier>)  [unwired: 9 in, 1 out]
            n316 = case shown="Default" w865 {
              tunnel: [w868 w872] -> w864
              tunnel: w863 -> [_ w872]
              tunnel: w862 -> [w871 _]
              frame Default {
                n317 = call-dynamic "Get Root Test.vi"("Test Event Storage in"=w871) -> ("Test"=w869:string)  [unwired: 8 in, 2 out]
                n318 = Bundle By Name(cluster=errorcluster {"status"=TRUE, "code"=7002, "source"=""} ("Test"), "status"=TRUE, "source"=w869, "code"=7002) -> (w868:errorcluster)
              }
              frame "Unknown", "Pass", "Skip" {
              }
            }
            n319 = Send Notification(notification=w864, notifier=w860) -> (error out=w857:errorcluster)  [unwired: 1 in, 1 out]
            n320 = call <vilib>:"Clear Errors.vi"("error in (no error)"=w857) -> ("error out"=w859:errorcluster)  [unwired: 5 in, 1 out]
            n321 = call "Message Event Global.vi"("error in (no error)"=w859, "Clear (F)"=TRUE) -> ()  [unwired: 6 in, 4 out]
          }
          frame Error {
            # "Ignore if message is not of\ntype \"Complete Suite\""
          }
        }
        n322 = Merge Errors(w846) -> (w845:errorcluster)
        n323 = call <vilib>:"Add State(s) to Queue__jki_lib_state_machine.vi"("State(s) in (\"\")"=w856) -> ("States Out"=w855:string)  [unwired: 14 in]
      }
      frame "Test: Reset" {
        w876 = Test_State."Unknown"  # State
        w879 = refnum<class "Test Event Storage.lvclass"> refnum  # Storage
        n324 = Bundle By Name(cluster=w878, "Complete"=FALSE ("UI Needs Update"), "Final State"=w876, "State"=w876, "Update Delay"=u32 100, "Storage"=w879) -> (w880:T8)
        n325 = call <vilib>:"Add State(s) to Queue__jki_lib_state_machine.vi"("State(s) in Front (\"\")"="UI: Clear", "State(s) in (\"\")"=w883) -> ("States Out"=w882:string)  [unwired: 13 in]
      }
      frame "Test: Reset?" {
        n326 = Unbundle By Name(w888) -> ("Complete"=w887:bool)
        n327 = Select(t="Test: Reset", s=w887, f="") -> (s? t:f=w885:string)
        n328 = call <vilib>:"Add State(s) to Queue__jki_lib_state_machine.vi"("State(s) in Front (\"\")"=w885, "State(s) in (\"\")"=w892) -> ("States Out"=w891:string)  [unwired: 13 in]
      }
      frame "Test: Set Running" {
        n329 = Bundle By Name(cluster=w896, "Running"=TRUE) -> (w895:T8)
        n330 = call <vilib>:"Add State(s) to Queue__jki_lib_state_machine.vi"("State(s) in (\"\")"=w899) -> ("States Out"=w898:string)  [unwired: 14 in]
      }
      frame "Test: Exit?" {
        n331 = Unbundle By Name(w904) -> ("Interactive"=w906:bool)
        n332 = Select(t="Reset Final Error", s=w906, f="Macro: Exit") -> (s? t:f=w905:string)
        n333 = call <vilib>:"Add State(s) to Queue__jki_lib_state_machine.vi"("State(s) in Front (\"\")"=w905, "State(s) in (\"\")"=w909) -> ("States Out"=w908:string)  [unwired: 13 in]
      }
      frame "Test: Export Report" {
        n334 = Unbundle By Name(w917) -> ("Storage"=w916:refnum<class "Test Event Storage.lvclass">)
        n335 = call "Read Test Report.vi"("Basic Test Manager"=w915) -> ("Test Report"=w913:refnum<class "Test Report.lvclass">, "Basic Test Manager"=w914:refnum<class "Basic Test Manager.lvclass">)  [unwired: 9 in]
        n336 = call-dynamic "isReporting.vi"("Test Report in"=w913) -> ("Exporting?"=w912:bool, "Test Report out"=w910:refnum<class "Test Report.lvclass">)  [unwired: 8 in, 1 out]
        n337 = case shown="True" w912 {
          tunnel: w914 -> [w925 _]
          tunnel: w919 -> [w924 w926]
          tunnel: [w923 w926] -> w918
          tunnel: w916 -> [w922 _]
          tunnel: w910 -> [_ _]
          frame False {
            n338 = call "Export Report.vi"("error in (no error)"=w924, "Storage"=w922, "Basic Test Manager in"=w925) -> ("error out"=w923:errorcluster)  [unwired: 7 in, 1 out]
          }
          frame True {
          }
        }
        n339 = call <vilib>:"Add State(s) to Queue__jki_lib_state_machine.vi"("State(s) in (\"\")"=w921) -> ("States Out"=w920:string)  [unwired: 14 in]
      }
      frame "Test: Local Report" {
        n340 = Unbundle By Name(w933) -> ("Report Event"=w938:refnum<user-event>)
        n341 = Unbundle By Name(w933) -> ("Storage"=w930:refnum<class "Test Event Storage.lvclass">)
        n342 = Unbundle By Name(w939) -> ("local"=w940:refnum<event-registration>)
        n343 = register-events(reference=w940, error in=w928, w938) -> (error out=w941:errorcluster)  [unwired: 1 out]
        n344 = call "Create EventReport.vi"("error in (no error)"=w941, "Report Event"=w938) -> ("error out"=w929:errorcluster, "Test Report.Event out"=w932:refnum<class "Test Report.Event.lvclass">)  [unwired: 8 in]
        n345 = call "Generate Results.vi"("error in (no error)"=w929, "Storage"=w930, "Basic Test Manager in"=w927) -> ("error out"=w936:errorcluster, "Test Result"=w934:refnum<class "Test Result.lvclass">)  [unwired: 6 in, 1 out]
        n346 = call "Write Test Result.vi"("error in (no error)"=w936, "Test Result"=w934, "Test Report in"=w932) -> ("error out"=w935:errorcluster, "Test Report out"=w937:refnum<class "Test Report.Event.lvclass">)  [unwired: 7 in]
        n347 = call-dynamic "Export.vi"("error in (no error)"=w935, "Test Report in"=w937) -> ("error out"=w931:errorcluster)  [unwired: 8 in, 1 out]
        n348 = call <vilib>:"Add State(s) to Queue__jki_lib_state_machine.vi"("State(s) in (\"\")"=w943) -> ("States Out"=w942:string)  [unwired: 14 in]
      }
      frame "Test: Publish Test Result" {
        n349 = Unbundle By Name(w955) -> ("Storage"=w954:refnum<class "Test Event Storage.lvclass">, "Message"=w946:refnum<class "TestManagerMsg.lvclass">)
        n350 = call "Generate Results.vi"("error in (no error)"=w952, "Storage"=w954, "Basic Test Manager in"=w953) -> ("error out"=w949:errorcluster, "Test Result"=w950:refnum<class "Test Result.lvclass">, "Basic Test Manager out"=w951:refnum<class "Basic Test Manager.lvclass">)  [unwired: 6 in]
        n351 = call "Read Test Suite Result.vi"("error in (no error)"=w949, "Basic Test Manager in"=w951) -> ("error out"=w947:errorcluster, "Test Suite Result"=w945:refnum<user-event>)  [unwired: 7 in, 1 out]
        n352 = Generate User Event(user event=w945, event data cluster=w950, error in=w947) -> (error out=w948:errorcluster)  [unwired: 1 in, 1 out]
        n353 = disable-structure shown="Disabled" {
          disable-tunnel: w946 -> [_ _]
          disable-tunnel: w945 -> [w958 _]
          frame Disabled {
            n354 = Generate User Event(user event=w958) -> ()  [unwired: 3 in, 2 out]
          }
          frame Enabled {
          }
        }
        n355 = call <vilib>:"Add State(s) to Queue__jki_lib_state_machine.vi"("State(s) in (\"\")"=w957) -> ("States Out"=w956:string)  [unwired: 14 in]
      }
      frame "Test: Export?" {
        n356 = Unbundle By Name(w984) -> ("Storage"=w979:refnum<class "Test Event Storage.lvclass">)
        n357 = call-dynamic "Get All Test Registrations.vi"("error in (no error)"=w977, "Test Event Storage in"=w979) -> ("error out"=w976:errorcluster, "Test Registrations"=w975:T3[], "Test Event Storage out"=w978:refnum<class "Test Event Storage.lvclass">)  [unwired: 5 in, 2 out]
        n358 = Index Array(array=w975) -> (element=w974:T3)  [unwired: 1 in]
        n359 = case shown="\"JUnit\"" w962 {
          tunnel: ["*.txt" ("pattern (all files)") "*.xml" ("pattern (all files)")] -> w965
          tunnel: ["Text file" ("pattern label") "XML file" ("pattern label")] -> w964
          frame Default {
          }
          frame "JUnit" {
          }
        }
        n360 = Unbundle By Name(w974) -> ("Test Registration.Name"=w967:string)
        n361 = call-poly <userlib>:"Strip Path Extension__ogtk.vi"("path"=w967) -> ("root"=w966:string)  [unwired: 1 out]
        n362 = disable-structure shown="Default" {
          disable-tunnel: [w997 _] -> w982
          disable-tunnel: "Select Report File" ("prompt") -> [w996 _]
          disable-tunnel: "Export" ("button label") -> [w995 _]
          disable-tunnel: w976 -> [w994 _]
          disable-tunnel: [w993 _] -> w973
          disable-tunnel: [w992 _] -> w972
          disable-tunnel: w966 -> [w991 _]
          disable-tunnel: w965 -> [w990 _]
          disable-tunnel: w964 -> [w989 _]
          disable-tunnel: [w988 _] -> w963
          frame condition #0 (active) {
            n363 = call "File Dialog"("prompt"=w996, "button label"=w995, "default name"=w991, "error in"=w994, "pattern (all files)"=w990, "pattern label"=w989) -> ("selected path"=w988:path, "exists"=w993:bool, "cancelled"=w997:bool, "error out"=w992:errorcluster)  [unwired: 6 in]
          }
          frame condition #1 {
          }
        }
        n364 = case shown="\"JUnit\"" w962 {
          tunnel: w963 -> [w999 w1001]
          tunnel: [w998 w1000] -> w961
          frame Default {
            n365 = call "Create DefaultReport.vi"("Report Path"=w999) -> ("Test Report.Default out"=w998:refnum<class "Test Report.Default.lvclass">)  [unwired: 9 in, 1 out]
          }
          frame "JUnit" {
            n366 = call "Create JUnit Report.vi"("Report Path"=w1001) -> ("Test Report.JUnit out"=w1000:refnum<class "Test Report.JUnit.lvclass">)  [unwired: 9 in, 1 out]
          }
        }
        n367 = case shown="True" w973 {
          tunnel: w963 -> [_ w1010]
          tunnel: w972 -> [w1006 w1007]
          tunnel: [w1006 w1009] -> w960
          tunnel: [_ w1008] -> w971
          frame False {
          }
          frame True {
            n368 = call "Overwrite Dialog.vi"("error in (no error)"=w1007, "Path"=w1010) -> ("error out"=w1009:errorcluster, "Cancelled?"=w1008:bool)  [unwired: 8 in]
          }
        }
        n369 = call "Write Test Report.vi"("Test Report"=w961, "Basic Test Manager"=w970) -> ("Basic Test Manager"=w969:refnum<class "Basic Test Manager.lvclass">)  [unwired: 9 in]
        n370 = call-dynamic "isReporting.vi"("Test Report in"=w961) -> ("Exporting?"=w968:bool)  [unwired: 8 in, 2 out]
        n371 = Compound Arithmetic op=OR(w968, w971, w982, w960) -> (w983:bool)
        n372 = case shown="False" w983 {
          tunnel: w969 -> [w1014 _]
          tunnel: w976 -> [w1013 w1015]
          tunnel: [w1012 w1015] -> w985
          tunnel: w978 -> [w1011 _]
          frame False {
            n373 = call "Export Report.vi"("error in (no error)"=w1013, "Storage"=w1011, "Basic Test Manager in"=w1014) -> ("error out"=w1012:errorcluster)  [unwired: 7 in, 1 out]
          }
          frame True {
          }
        }
        n374 = call <vilib>:"Add State(s) to Queue__jki_lib_state_machine.vi"("State(s) in (\"\")"=w987) -> ("States Out"=w986:string)  [unwired: 14 in]
      }
      frame "Test: Complete" {
        # "First time we're called and we didn't pass?\n    Yes: Hide Passed Tests\n    No: Don't change it's value"
        n375 = Unbundle By Name(w1031) -> ("State"=w1026:T7, "Hide Passed Tests"=w1021:bool, "Start Time"=w1017:timestamp)
        n376 = First Call?() -> (First Call?: T/F=w1028:bool)
        n377 = Get Date/Time In Seconds() -> (seconds since 1Jan1904=w1018:timestamp)
        n378 = Not Equal?(x=w1026, y=Test_State."Pass" ("State")) -> (x != y?=w1027:bool)
        n379 = And(x=w1028, y=w1027) -> (x .and. y?=w1024:bool)
        n380 = Subtract(x=w1018, y=w1017) -> (x-y=→"Processing Time (s)":dbl)
        n381 = Select(t=TRUE, s=w1024, f=w1021) -> (s? t:f=w1022:bool)
        n382 = Bundle By Name(cluster=w1031, "Complete"=TRUE ("UI Needs Update"), "Final State"=w1026, "Running"=FALSE, "Hide Passed Tests"=w1022, "Start Time"=timestamp(0 s since 1904-01-01)) -> (w1032:T8)
        n383 = call <vilib>:"Add State(s) to Queue__jki_lib_state_machine.vi"("State(s) in (\"\")"=w1035) -> ("States Out"=w1034:string)  [unwired: 14 in]
      }
    }
  }
  "error out" <- w1
  "Test Manager out" <- "Test Manager"
